vi "VI Doc Editor.vi"(11 "VI Path in":path) -> (0 "OK out":bool, 3 "dup VI Path in":path)   [LabVIEW 2014]
doc: "::: VI Helpeks :::\nCopyright (c) 2000-2026 Konstantin Shifershteyn. All rights reserved."
uses:
  <vilib>/event_ctls.llb/lveventtype.ctl
  <vilib>/Utility/miscctls.llb/LVPointTypeDef.ctl
  <vilib>/picture/picture.llb/imagedata.ctl
  <vilib>/Utility/cursorutil.llb/Set Cursor (Icon Pict).vi
  _VIH Support Library.llb/VIH Utility - APP - Is Value Changed (I32).vi
  _VIH Support Library.llb/VIH Utility - MENU - Create Menu (String).vi
panel:
  out "Conpane Image":picture caption="Connector Pane Image"
  in  "Ctrl Tree":string[](tree) caption="Control Tree"
  in  "Sort":cluster{"Column":i32, "Reverse":bool}
  in  "App Refnum":refnum<vi>
  in  "Good VI":bool
  in  "Changed":bool
  in  "VI Path":path
  in  "Tab Control":enum32{"VI Properties", "Control Properties"}(tab)
  out "VI Version":string caption="Source version"
  in  "VI Cust Title":bool caption="Same as VI Name"
  in  "VI Title":string caption="VI Front Panel Title"
  out "VI Icon":picture
  in  "VI Help Path":path caption="Help Path"
  in  "VI Help Tag":string caption="Help Tag"
  in  "VI Description":string
  in  "VI Help Use Url":i16(ring) caption="Help Used" items=["Local Help File", "Web-based Help"]
  in  "VI Help Url":string caption="Help URL"
  out "Ctrl Icon":picture caption="Terminal icon"
  in  "Ctrl Tooltip":string caption="Tip"
  in  "Ctrl Description":string caption="Description"
  in  "Ctrl Caption":string caption="Caption"
  out "Ctrl Label":string="Control label" caption="Control Label"
  in  "ConpaneMenuActive":bool
  in  "%OpenVI":bool caption="Open VI"
  in  "%Apply&Save":bool caption="Apply and Save VI"
  in  "%Apply":bool caption="Apply to VI"
  in  "%EXIT":bool caption="Exit"
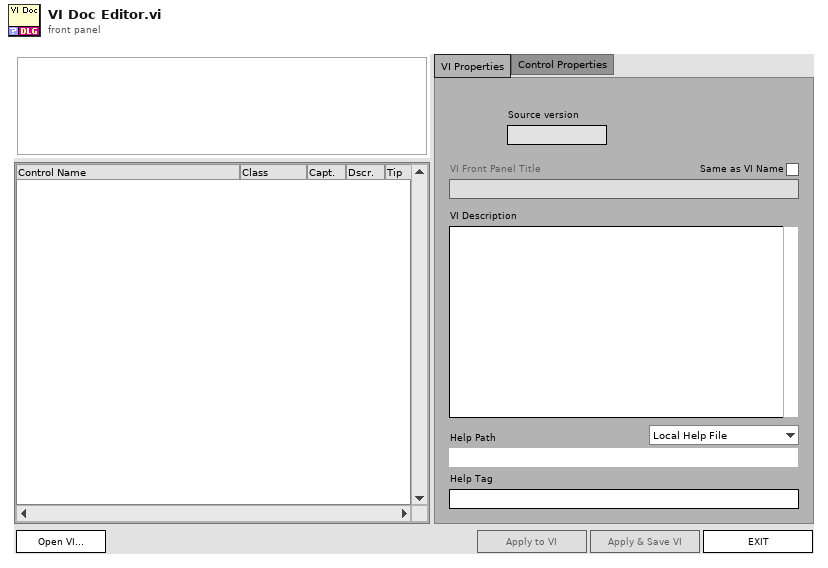
[diagram p1: front panel]
types:
  T1 = typedef "lveventtype.ctl" = enum32{"Null", "Timeout", "Annotation Menu Selection", "Annotation Menu Selection?", "App Instance Close", "App Instance Close?", "Autoscale Range Change", "Bookmark Info Change", "Cell Edit", "Cell Edit?", "Cursor Grab", "Cursor Grab?", "Cursor Menu Selection", "Cursor Menu Selection?", "Cursor Move", "Cursor Release", "Data Change", "Direction Change", "Display State Change", "Drag Ended", "Drag Enter", "Drag Leave", "Drag Over", "Drag Source Update", "Drag Starting", "Drag Starting?", "Drop", "Exec State Change", "Key Down", "Key Down?", "Key Repeat", "Key Repeat?", "Key Up", "Listbox Double Click", "Menu Activation?", "Menu Selection (App)", "Menu Selection? (App)", "Menu Selection (User)", "Mouse Down", "Mouse Down?", "Mouse Enter", "Mouse Leave", "Mouse Move", "Mouse Up", "Mouse Wheel", "NI Security User Change (App)", "Pane Size", "Panel Close", "Panel Close?", "Panel Resize", "Plot Attribute Change", "Scale Range Change", "Shortcut Menu Activation?", "Shortcut Menu Selection (App)", "Shortcut Menu Selection? (App)", "Shortcut Menu Selection (User)", "Tree Double Click", "Tree Drag", "Tree Drag?", "Tree Drop", "Tree Drop?", "Tree Item Close", "Tree Item Close?", "Tree Item Open", "Tree Item Open?", "User Event", "Value Change"}
  T2 = enum16{"nop", "Init", "get index", "get symbols"}
  T3 = typedef "LVPointTypeDef.ctl" = cluster{"Horizontal":i16, "Vertical":i16}
  T4 = cluster{"Width":i16, "Style":enum32{"Solid", "Dash", "Dot", "DashDot", "DashDotDot"}}
  T5 = enum16{"Apply", "ApplySave", "Continue", "Cancel"}
  T6 = typedef "imagedata.ctl" = cluster{"image type":i32, "image depth":i32, "image":u8[], "mask":u8[], "colors":u32[], "Rectangle":cluster{"left":i16, "top":i16, "right":i16, "bottom":i16}}
  T7 = cluster{"VI Reference":refnum<vi>, "Changed":bool, "Description":string, "Help.Path":path, "Help.Tag":string, "CustomTitle":bool, "Title":string, "Icon":T6, "Help.UseWebUrl":bool, "Help.WebUrl":string}
  T8 = enum32{"Bad", "Idle", "Run top level", "Running"}
  T9 = enum32{"Invalid", "Default", "Floating", "Floating/Auto-Hide", "Modal"}
  T10 = enum8{"Enabled", "Disabled", "Disabled and Grayed Out"}
  T11 = typedef "LVRectTypeDef.ctl" = cluster{"Left":i16, "Top":i16, "Right":i16, "Bottom":i16}
  T12 = typedef "LVPoint32TypeDef.ctl" = cluster{"Horizontal":i32, "Vertical":i32}
  T13 = typedef "LVMouseTypeDef.ctl" = cluster{"Mouse Position":cluster{"X":i32, "Y":i32}, "Mouse Modifiers":cluster{"Button Down":bool, "Shift Mod":bool, "Menu Mod":bool, "Option Mod":bool}}
  T14 = cluster{"Button Down":bool, "Shift Mod":bool, "Menu Mod":bool, "Option Mod":bool}
  T15 = cluster{"Ctrl ID":string, "Conpane Idx":i32, "Bounds":cluster{"X0":i32, "Y0":i32, "X1":i32, "Y1":i32}}[]
  T16 = cluster{"Ctrl ID":string, "Conpane Idx":i32, "Bounds":cluster{"X0":i32, "Y0":i32, "X1":i32, "Y1":i32}}
  T17 = typedef "VIH Project Tree Typedef - Tree Refnum.ctl" = refnum<vi>
  T18 = typedef "VIH - VI Doc Editor #2 Typedef - Info Cluster.ctl" = cluster{"Control Label":string, "Class Name":string, "Indicator":bool, "Error Cluster":bool, "Tree Tag":string, "Control ID":string, "Conpane Idx":i32, "Ctl Refnum":refnum<vi>, "Ctl Caption":string, "Ctl Description":string, "Ctl Tooltip":string, "Page Refnum":refnum<vi>}
  T19 = cluster{"Has Caption":bool, "Caption":string, "Description":string, "Tip Strip":string}
  T20 = cluster{"left":i16, "top":i16, "right":i16, "bottom":i16}
  T21 = typedef "LVBoundsTypeDef.ctl" = cluster{"Width":u32, "Height":u32}
  T22 = cluster{"image":picture, "Rectangle":cluster{"left":i16, "top":i16, "right":i16, "bottom":i16}}
  T23 = typedef "VIH HelpGen Typedef - Control Terminal Attributes Cluster.ctl" = cluster{"Conpane Idx":i32, "Control":bool, "Wire Rule":enum16{"Invalid Wire Rule", "Required", "Recommended", "Optional", "Dynamic Dispatch"}}
  T24 = cluster{"Description":string, "Help.Path":path, "Help.Tag":string, "CustomTitle":bool, "Title":string, "Help.UseWebUrl":bool, "Help.WebUrl":string}
  T25 = cluster{"Ctl Caption":string, "Ctl Description":string, "Ctl Tooltip":string}
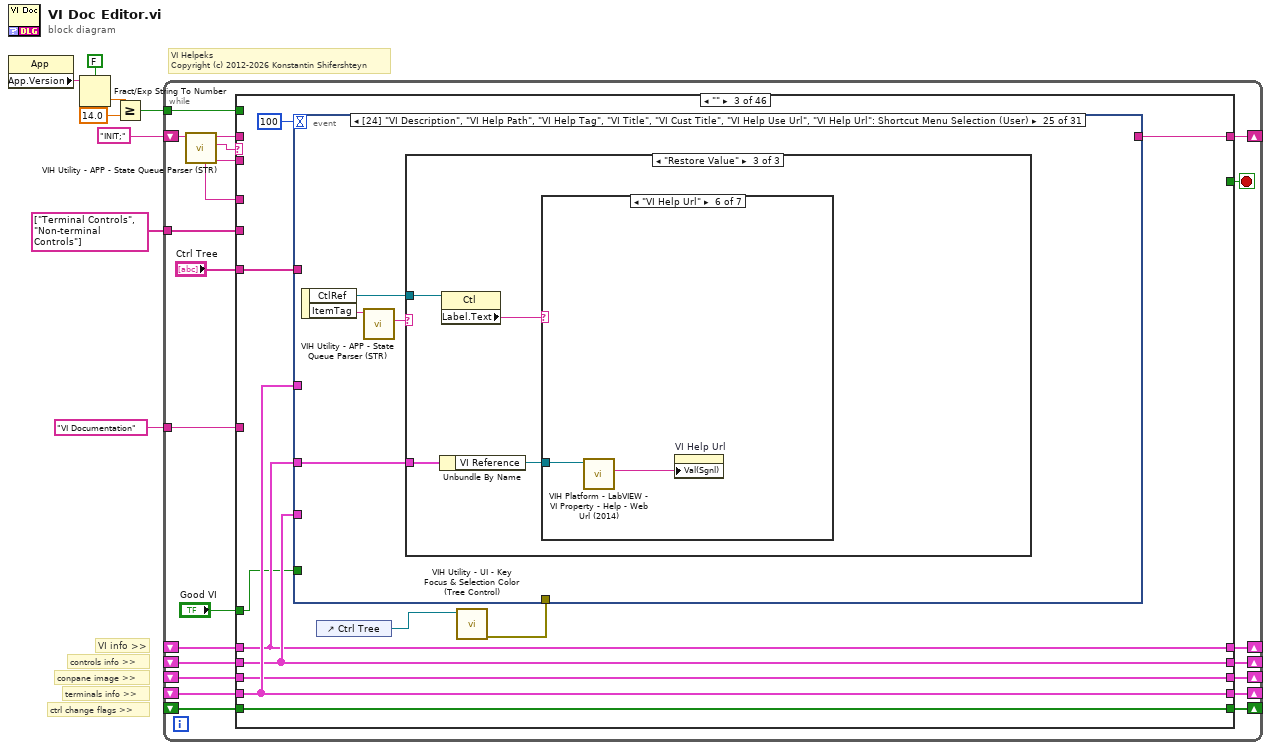
[diagram p0: block diagram]
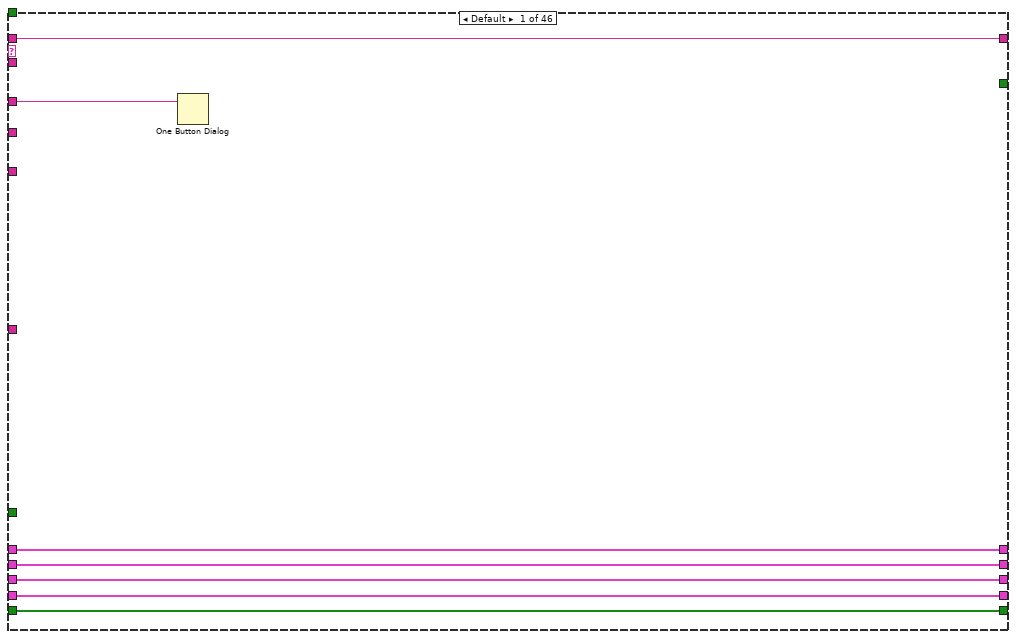
[diagram p2: hidden frame]
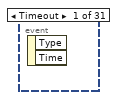
[diagram p4: hidden frame]
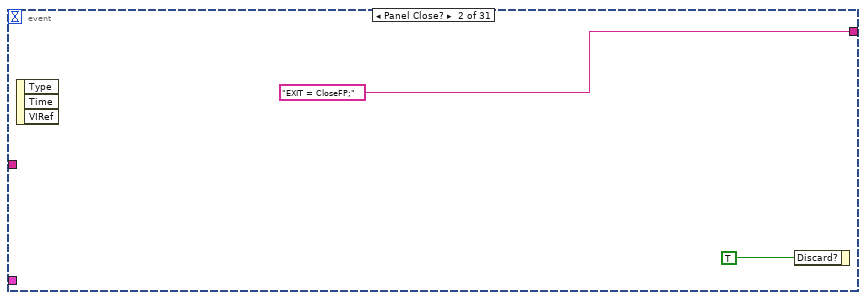
[diagram p5: hidden frame]
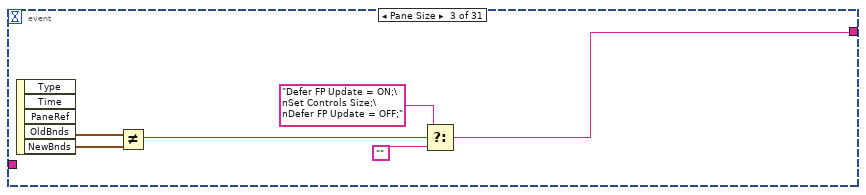
[diagram p6: hidden frame]
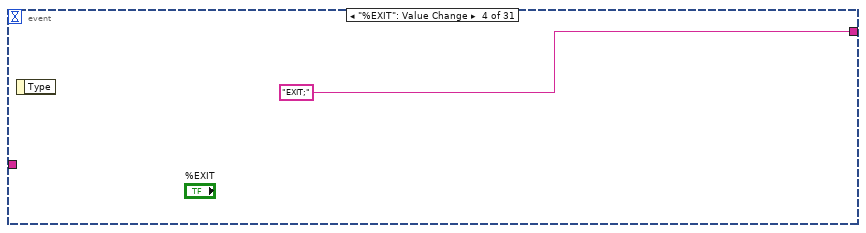
[diagram p7: hidden frame]
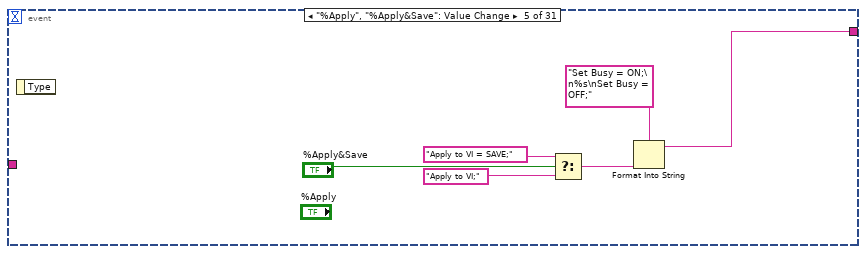
[diagram p8: hidden frame]
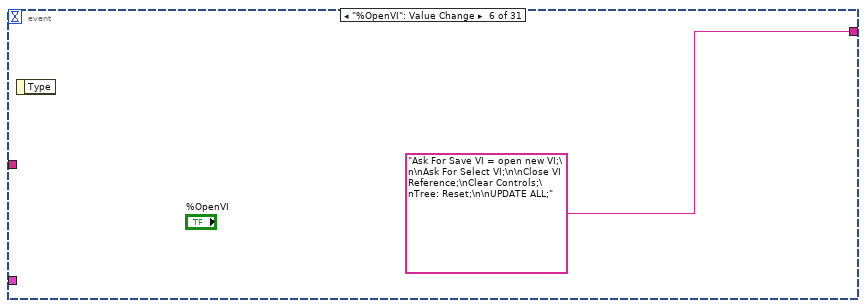
[diagram p9: hidden frame]
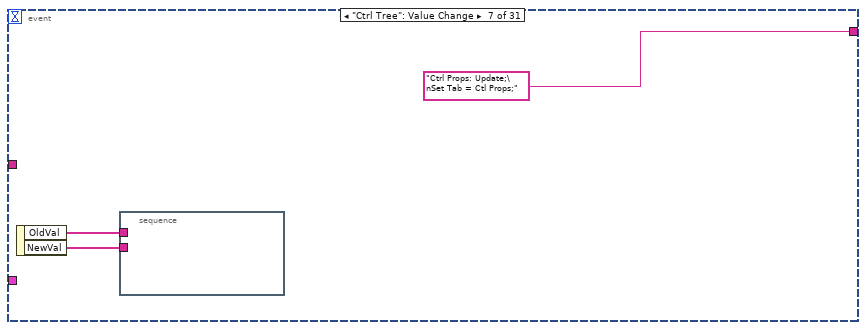
[diagram p10: hidden frame]
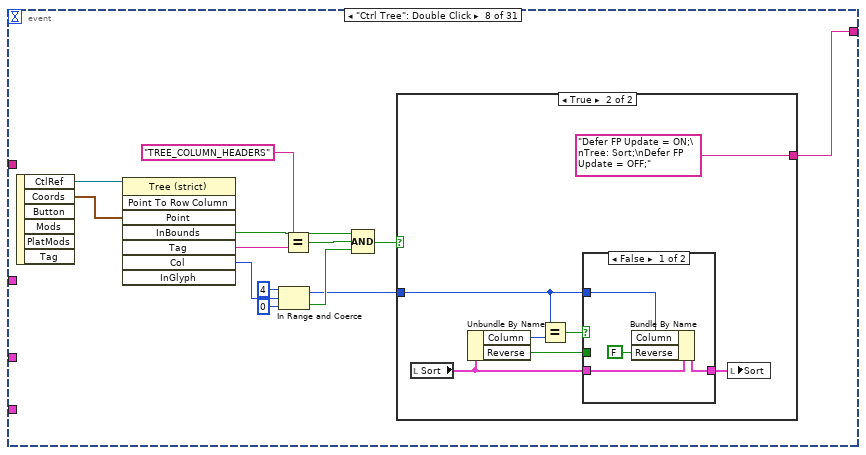
[diagram p11: hidden frame]
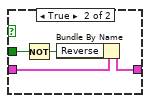
[diagram p13: hidden frame]
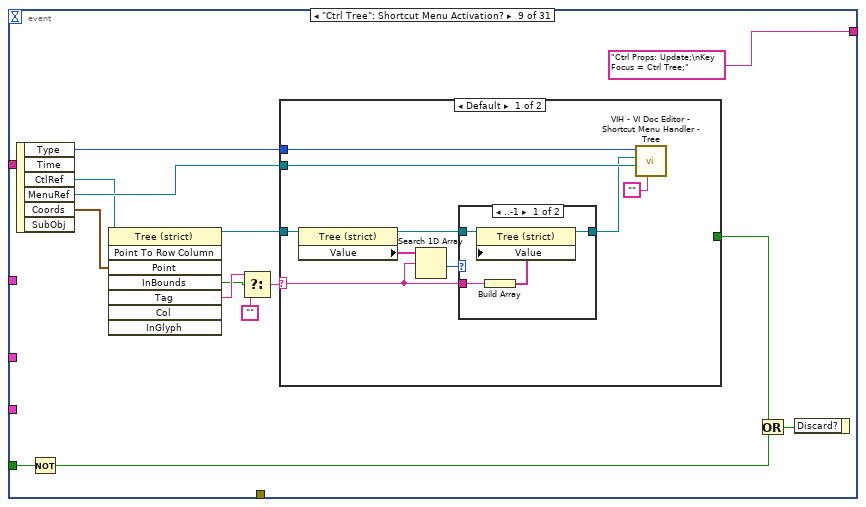
[diagram p14: hidden frame]
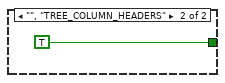
[diagram p16: hidden frame]
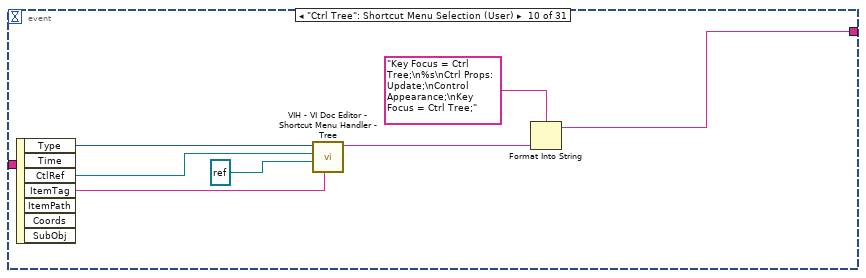
[diagram p17: hidden frame]
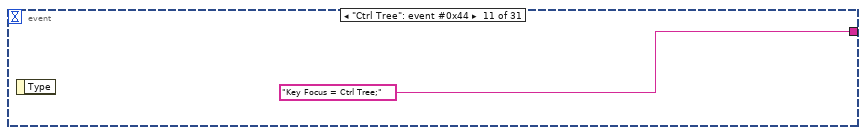
[diagram p18: hidden frame]
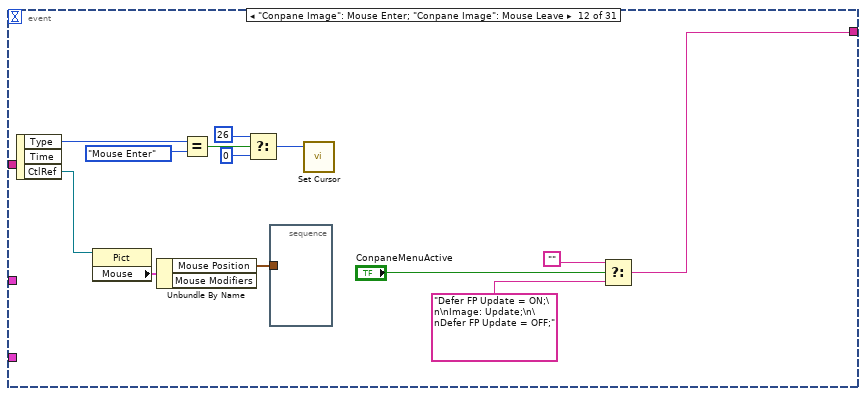
[diagram p19: hidden frame]
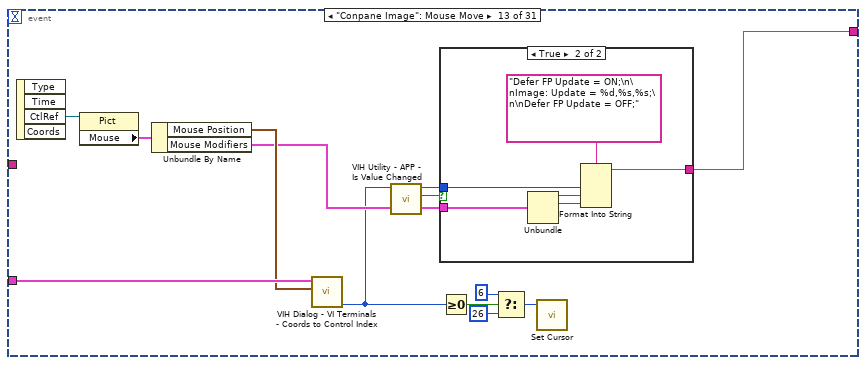
[diagram p20: hidden frame]
diagram:
  # "VI Helpeks\nCopyright (c) 2012-2026 Konstantin Shifershteyn"
  # "ctrl change flags >>"
  # "VI info >>"
  # "terminals info >>"
  # "conpane image >>"
  # "controls info >>"
  n1 = property class="App"() -> ("App.Version"=w6:string)  [unwired: 2 in, 2 out]
  n2 = Fract/Exp String To Number(use system decimal point (T)=FALSE, string=w6) -> (number=w4:dbl)  [unwired: 2 in, 1 out]
  n3 = Greater Or Equal?(x=w4, y=14.0) -> (x >= y?=w2:bool)
  n4 = while {
    shift-right: [w27] -> _
    shift-left: "INIT;" -> [w29]
    shift-right: [w22] -> _
    shift-left: _ -> [w21]
    shift-right: [w20] -> _
    shift-left: _ -> [w19]
    shift-right: [w18] -> _
    shift-left: _ -> [w17]
    tunnel: "VI Documentation" -> [w16]
    shift-right: [w15] -> _
    shift-left: _ -> [w14]
    shift-right: [w13] -> _
    shift-left: _ -> [w12]
    tunnel: w2 -> [w10]
    tunnel: string[] ["Terminal Controls", "Non-terminal Controls"] -> [w9]
    stop <- w23 stop-if-true
    n5 = call "VIH Utility - APP - State Queue Parser (STR).vi"("input queue"=w29) -> ("state parameters"=w25:string, "state"=w30:string, "remained queue"=w28:string, "complete state specifier"=w26:string)  [unwired: 5 in]
    n6 = case shown="\"\"" w30 {
      tunnel: w28 -> [w37 w43 _ w430 w466 _ w504 w512 w519 w528 w545 w587 w625 w633 w682 w685 w704 w709 w729 w760 w766 w800 w819 w861 w894 w935 w970 w997 w1021 w1028 w1035 w1042 w1055 w1108 w1112 w1158 w1188 w1208 w1229 w1250 w1262 w1318 w1347 w1367 w1389 w1556]
      tunnel: [w37 w43 w51 w427 w463 w468 w504 w512 w519 w528 w545 w587 w625 w633 w682 w684 w704 w708 w730 w760 w767 w800 w819 w861 w894 w935 w970 w997 w1021 w1028 w1035 w1042 w1055 w1108 w1112 w1158 w1188 w1202 w1225 w1250 w1262 w1309 w1346 w1367 w1378 w1550] -> w27
      tunnel: w26 -> [w36 _ _ _ _ _ _ _ _ _ _ _ _ _ _ _ _ _ _ _ _ _ _ _ _ _ _ _ _ _ _ _ _ _ _ _ _ _ _ _ _ _ _ _ _ _]
      tunnel: w25 -> [_ _ _ _ _ w467 w485 _ w518 w527 w544 _ _ w631 _ w689 _ _ w731 _ _ _ _ _ _ _ _ w982 _ _ _ _ w1047 _ _ _ _ _ w1221 _ w1258 w1305 w1342 _ w1380 w1547]
      tunnel: "Ctrl Tree" -> [_ _ w45 _ _ _ _ _ _ _ _ _ _ _ _ _ _ _ _ _ _ _ _ _ _ _ _ _ _ _ _ w1039 w1045 _ _ _ _ _ _ _ w1257 w1320 _ _ _ _]
      tunnel: [_ _ _ _ _ _ TRUE _ _ _ _ _ _ _ _ _ _ _ _ _ _ _ _ _ _ _ _ _ _ _ _ _ _ _ _ _ _ _ _ _ _ _ _ _ _ _] -> w23
      tunnel: [w35 w42 w50 w429 w465 w474 w501 w511 w517 w524 w540 w586 w624 w632 w681 w694 w703 w719 w737 w759 w783 w799 w818 w838 w893 w916 w968 w995 w1019 w1026 w1033 w1041 w1054 w1107 w1116 w1166 w1187 w1207 w1228 w1249 w1261 w1317 w1353 w1366 w1388 w1555] -> w22
      tunnel: w21 -> [w35 w42 w50 w429 w465 w474 w501 w511 w517 w524 w540 w586 w624 w632 w681 w694 w703 w719 w737 w759 w783 w799 w818 w838 w893 _ w968 w995 w1019 w1026 w1033 w1041 w1054 w1107 w1116 w1166 w1187 w1207 w1228 w1249 w1261 w1317 w1353 w1366 w1388 w1555]
      tunnel: [w34 w41 w49 w428 w464 w473 w500 w510 w516 w523 w539 w585 w623 w630 w680 w693 w702 w718 w736 w758 w782 w798 w817 w834 w892 w909 w969 w996 w1020 w1025 w1032 w1040 w1053 w1106 w1115 w1165 w1186 w1206 w1227 w1248 w1260 w1316 w1352 w1365 w1387 w1554] -> w20
      tunnel: w19 -> [w34 w41 w49 w428 w464 w473 w500 w510 w516 w523 w539 w585 w623 w630 w680 w693 w702 w718 w736 w758 w782 w798 w817 _ w892 w909 w969 w996 w1020 w1025 w1032 w1040 w1053 w1106 w1115 w1165 w1186 w1206 w1227 w1248 w1260 w1316 w1352 w1365 w1387 w1554]
      tunnel: [w33 w40 w48 w426 w462 w472 w497 w509 w515 w522 w534 w584 w622 w629 w679 w692 w701 w717 w735 w757 w781 w796 w816 w837 w891 w918 w967 w994 w1018 w1024 w1031 w1038 w1050 w1105 w1114 w1164 w1185 w1205 w1226 w1247 w1251 w1315 w1348 w1364 w1382 w1552] -> w18
      tunnel: w17 -> [w33 w40 w48 w426 w462 w472 w497 w509 w515 w522 w534 w584 w622 w629 w679 w692 w701 w717 w735 w757 w781 w796 w816 w837 w891 _ w967 w994 w1018 w1024 w1031 w1038 w1050 w1105 w1114 w1164 w1185 w1205 w1226 w1247 w1255 w1315 w1350 w1364 w1382 w1552]
      tunnel: w16 -> [_ _ _ _ _ _ w499 _ _ _ _ w583 _ _ _ _ _ _ w732 _ _ w797 _ _ _ _ _ _ _ _ _ _ _ _ _ _ _ _ _ _ _ _ _ _ _ _]
      tunnel: [w32 w39 w46 w423 w461 w471 w496 w508 w514 w521 w533 w580 w621 w628 w678 w691 w700 w716 w734 w756 w780 w793 w804 w841 w890 w924 w965 w993 w1017 w1023 w1030 w1037 w1052 w1104 w1110 w1157 w1184 w1203 w1223 w1246 w1259 w1314 w1351 w1363 w1384 w1553] -> w15
      tunnel: w14 -> [w32 w39 w46 w423 w461 w471 w496 w508 w514 w521 w533 w580 w621 w628 w678 w691 w700 w716 w734 w756 _ w793 w804 w841 w890 w924 w965 w993 w1017 w1023 w1030 w1037 w1052 w1104 w1111 w1156 w1184 w1204 w1220 w1246 w1259 w1314 w1351 w1363 w1384 w1553]
      tunnel: [w31 w38 w47 w422 w460 w470 w495 w507 w513 w520 w532 w579 w616 w627 w677 w690 w699 w715 w733 w755 w779 w791 w815 w839 w889 w910 w962 w992 w1016 w1022 w1029 w1036 w1048 w1103 w1113 w1159 w1181 w1200 w1224 w1245 w1252 w1307 w1345 w1362 w1381 w1551] -> w13
      tunnel: w12 -> [w31 w38 w47 w422 w460 w470 w495 w507 w513 w520 w532 w579 w616 w627 w677 w690 w699 w715 w733 w755 w779 w791 w815 w839 w889 _ w962 w992 w1016 w1022 w1029 w1036 w1049 w1103 w1113 w1159 w1181 w1200 w1224 w1245 w1253 w1307 w1345 w1362 w1381 w1551]
      tunnel: "Good VI" -> [_ _ w44 _ _ _ _ _ _ _ _ w574 _ _ _ _ _ _ _ _ _ _ _ w833 _ _ _ _ _ _ _ _ _ _ _ _ w1173 _ _ _ _ w1304 _ _ _ _]
      tunnel: w10 -> [_ _ _ w406 _ _ _ _ _ _ _ _ _ _ _ _ _ _ _ _ _ _ _ _ _ _ _ _ _ _ _ _ _ _ _ _ w1167 _ _ _ _ _ _ _ _ _]
      tunnel: w9 -> [_ _ _ _ _ _ _ _ _ _ _ _ _ _ _ _ _ _ _ _ _ _ _ _ _ w895 w960 w976 _ _ _ _ _ _ _ _ _ _ _ _ _ _ _ _ _ _]
      frame Default {
        n7 = One Button Dialog(message=w36) -> ()  [unwired: 1 in, 1 out]
      }
      frame "#" {
      }
      frame "" {
        n8 = control-ref of="Ctrl Tree"() -> (w53:refnum<vi>)
        n9 = call "VIH Utility - UI - Key Focus & Selection Color (Tree Control).vi"("Tree Refnum"=w53) -> ("error out"=w52:errorcluster)  [unwired: 8 in, 2 out]
        n10 = event shown="[24] \"VI Description\", \"VI Help Path\", \"VI Help Tag\", \"VI Title\", \"VI Cust Title\", \"VI Help Use Url\", \"VI Help Url\": Shortcut Menu Selection (User)" {
          selector: _ -> [_ _ _ _ _ _ _ _ _ _ _ _ _ _ _ _ _ _ _ _ _ _ _ _ _ _ _ _ _ _ _]
          dyn-events: _ -> [_ _ _ _ _ _ _ _ _ _ _ _ _ _ _ _ _ _ _ _ _ _ _ _ _ _ _ _ _ _ _]
          timeout: 100 -> [_ _ _ _ _ _ _ _ _ _ _ _ _ _ _ _ _ _ _ _ _ _ _ _ _ _ _ _ _ _ _]
          tunnel: w52 -> [_ _ _ _ _ _ _ _ _ _ _ _ _ _ _ _ _ _ _ _ _ _ _ _ _ _ _ _ _ _ _]
          tunnel: [_ "EXIT = CloseFP;" w57 "EXIT;" w64 "Ask For Save VI = open new VI;\n\nAsk For Select VI;\n\nClose VI Reference;\nClear Controls;\nTree: Reset;\n\nUPDATE ALL;" "Ctrl Props: Update;\nSet Tab = Ctl Props;" w74 "Ctrl Props: Update;\nKey Focus = Ctrl Tree;" w132 "Key Focus = Ctrl Tree;" w142 w160 w176 w196 w263 w291 "Key Focus = Ctrl Tree;" "Image: Update;" "Image: Update;" w315 "VI Props: Apply;" _ _ _ w358 _ _ _ _ w395] -> w51
          tunnel: w50 -> [_ _ _ _ _ _ _ _ _ _ _ _ w164 w178 w199 w269 w288 w303 _ _ w316 _ _ _ _ _ _ _ _ _ _]
          tunnel: w48 -> [_ _ _ _ _ _ _ _ _ _ _ _ _ _ w190 w247 w275 _ _ _ _ _ _ _ _ _ _ w363 _ _ _]
          tunnel: w46 -> [_ _ _ _ _ _ _ _ _ _ _ _ _ _ _ _ _ _ _ _ _ _ _ _ w330 _ _ w367 _ _ _]
          tunnel: w45 -> [_ _ _ _ _ _ _ _ _ _ _ _ _ _ _ _ _ _ _ _ _ _ _ _ _ w360 _ w364 _ _ _]
          tunnel: w44 -> [_ _ _ _ _ _ _ _ w105 _ _ _ _ _ _ w244 _ _ _ _ _ _ _ _ _ _ _ _ _ _ _]
          event Timeout {
            n11 = event-data() -> ()  [unwired: 1 in, 2 out]
          }
          event Panel Close? {
            n12 = event-data() -> ()  [unwired: 1 in, 3 out]
            n13 = event-data("Discard?"=TRUE) -> ()  [unwired: 1 in, 1 out]
          }
          event Pane Size {
            n14 = event-data() -> ("OldBnds"=w62:T11, "NewBnds"=w61:T11)  [unwired: 1 in, 3 out]
            n15 = Not Equal?(x=w62, y=w61) -> (x != y?=w60:bool)
            n16 = Select(t="Defer FP Update = ON;\nSet Controls Size;\nDefer FP Update = OFF;", s=w60, f="") -> (s? t:f=w57:string)
          }
          event "%EXIT": Value Change {
            n17 = event-data() -> ()  [unwired: 1 in, 1 out]
          }
          event "%Apply", "%Apply&Save": Value Change {
            n18 = event-data() -> ()  [unwired: 1 in, 1 out]
            n19 = Select(t="Apply to VI = SAVE;", s="%Apply&Save", f="Apply to VI;") -> (s? t:f=w66:string)
            n20 = Format Into String(format string="Set Busy = ON;\n%s\nSet Busy = OFF;", w66) -> (resulting string=w64:string)  [unwired: 2 in, 1 out]
          }
          event "%OpenVI": Value Change {
            n21 = event-data() -> ()  [unwired: 1 in, 1 out]
          }
          event "Ctrl Tree": Value Change {
            n22 = event-data() -> ("OldVal"=w72:string[], "NewVal"=w71:string[])  [unwired: 1 in]
            n23 = stacked-sequence {
              tunnel: w72 -> [_]
              tunnel: w71 -> [_]
              frame #0 {
              }
            }
          }
          event "Ctrl Tree": Double Click {
            n24 = event-data() -> ("CtlRef"=w86:refnum<vi>, "Coords"=w85:T12)  [unwired: 1 in, 4 out]
            n25 = invoke class="Tree (strict)" method="Point To Row Column"(reference=w86, "Point"=w85) -> ("InBounds"=w79:bool, "Tag"=w81:string, "Col"=w84:i32)  [unwired: 6 in, 5 out]
            n26 = In Range and Coerce(upper limit=4, x=w84, lower limit=0) -> (coerced(x)=w75:i32, In Range?=w77:bool)
            n27 = Equal?(x="TREE_COLUMN_HEADERS", y=w81) -> (x = y?=w78:bool)
            n28 = Compound Arithmetic op=AND(w79, w78, w77) -> (w76:bool)
            n29 = case shown="True" w76 {
              tunnel: w75 -> [_ w88]
              tunnel: [_ "Defer FP Update = ON;\nTree: Sort;\nDefer FP Update = OFF;"] -> w74
              frame False {
              }
              frame True {
                n30 = local read "Sort"() -> (w92:cluster{"Column":i32, "Reverse":bool})
                n31 = Unbundle By Name(w92) -> ("Column"=w89:i32, "Reverse"=w91:bool)
                n32 = Equal?(x=w88, y=w89) -> (x = y?=w93:bool)
                n33 = case shown="False" w93 {
                  tunnel: w92 -> [w97 w101]
                  tunnel: w91 -> [_ w100]
                  tunnel: [w96 w99] -> w90
                  tunnel: w88 -> [w94 _]
                  frame False {
                    n34 = Bundle By Name(cluster=w97, "Column"=w94, "Reverse"=FALSE) -> (w96:cluster{"Column":i32, "Reverse":bool})
                  }
                  frame True {
                    n35 = Not(x=w100) -> (.not. x?=w98:bool)
                    n36 = Bundle By Name(cluster=w101, "Reverse"=w98) -> (w99:cluster{"Column":i32, "Reverse":bool})
                  }
                }
                n37 = local write "Sort"(w90) -> ()
              }
            }
          }
          event "Ctrl Tree": Shortcut Menu Activation? {
            n38 = event-data() -> ("Type"=w109:T1, "CtlRef"=w106:refnum<vi>, "MenuRef"=w108:refnum<k9>, "Coords"=w107:T12)  [unwired: 1 in, 2 out]
            n39 = Not(x=w105) -> (.not. x?=w104:bool)
            n40 = invoke class="Tree (strict)" method="Point To Row Column"(reference=w106, "Point"=w107) -> (reference out=w114:refnum<vi>, "InBounds"=w110:bool, "Tag"=w111:string)  [unwired: 6 in, 5 out]
            n41 = Select(t=w111, s=w110, f="") -> (s? t:f=w113:string)
            n42 = case shown="Default" w113 {
              selector: w113 -> [w119 _]
              tunnel: w108 -> [w120 _]
              tunnel: [_ TRUE] -> w103
              tunnel: w114 -> [w117 _]
              tunnel: w109 -> [w121 _]
              frame Default {
                n43 = property class="Tree (strict)"(reference=w117) -> (reference out=w122:refnum<vi>, "Value"=w124:string[])  [unwired: 1 in, 1 out]
                n44 = Search 1D Array(1D array=w124, element=w119) -> (index of element=w123:i32)  [unwired: 1 in]
                n45 = case shown="..-1" w123 {
                  tunnel: w122 -> [w128 w129]
                  tunnel: w119 -> [w127 _]
                  tunnel: [w125 w129] -> w116
                  frame ..-1 {
                    n46 = Build Array(w127) -> (w126:string[])
                    n47 = property class="Tree (strict)"(reference=w128, "Value"=w126) -> (reference out=w125:refnum<vi>)  [unwired: 1 in, 1 out]
                  }
                  frame 0.. {
                  }
                }
                n48 = call "VIH - VI Doc Editor - Shortcut Menu Handler - Tree.vi"("Menu Tag"="", "MenuRef"=w120, "Terminals Tree"=w116, "Event Type"=w121) -> ()  [unwired: 7 in, 1 out]
              }
              frame "", "TREE_COLUMN_HEADERS" {
              }
            }
            n49 = Or(x=w103, y=w104) -> (x .or. y?=w102:bool)
            n50 = event-data("Discard?"=w102) -> ()  [unwired: 1 in, 1 out]
          }
          event "Ctrl Tree": Shortcut Menu Selection (User) {
            n51 = event-data() -> ("Type"=w136:T1, "CtlRef"=w135:refnum<vi>, "ItemTag"=w134:string)  [unwired: 1 in, 4 out]
            n52 = call "VIH - VI Doc Editor - Shortcut Menu Handler - Tree.vi"("Menu Tag"=w134, "MenuRef"=refnum<k9> refnum, "Terminals Tree"=w135, "Event Type"=w136) -> ("States spec"=w133:string)  [unwired: 7 in]
            n53 = Format Into String(format string="Key Focus = Ctrl Tree;\n%s\nCtrl Props: Update;\nControl Appearance;\nKey Focus = Ctrl Tree;", w133) -> (resulting string=w132:string)  [unwired: 2 in, 1 out]
          }
          event "Ctrl Tree": event #0x44 {
            n54 = event-data() -> ()  [unwired: 1 in, 1 out]
          }
          event "Conpane Image": Mouse Enter; "Conpane Image": Mouse Leave {
            n55 = event-data() -> ("Type"=w151:T1, "CtlRef"=w140:refnum<vi>)  [unwired: 1 in, 1 out]
            n56 = property on="Property Node" class="Pict"(reference=w140) -> ("Mouse"=w141:T13)  [unwired: 1 in, 2 out]
            n57 = Unbundle By Name(w141) -> ("Mouse Position"=w139:cluster{"X":i32, "Y":i32})  [unwired: 1 out]
            n58 = Equal?(x=w151, y=lveventtype."Mouse Enter" ("Type")) -> (x = y?=w149:bool)
            n59 = Select(t=u16 26 ("icon"), s=w149, f=u16 0) -> (s? t:f=w146:u16)
            n60 = stacked-sequence {
              tunnel: w139 -> [_]
              frame #0 {
              }
            }
            n61 = call-poly <vilib>:"Set Cursor.vi"("icon"=w146) -> ()  [unwired: 9 in, 2 out]
            n62 = Select(t="", s="ConpaneMenuActive", f="Defer FP Update = ON;\n\nImage: Update;\n\nDefer FP Update = OFF;") -> (s? t:f=w142:string)
          }
          event "Conpane Image": Mouse Move {
            n63 = event-data() -> ("CtlRef"=w163:refnum<vi>)  [unwired: 1 in, 3 out]
            n64 = property on="Property Node" class="Pict"(reference=w163) -> ("Mouse"=w162:T13)  [unwired: 1 in, 2 out]
            n65 = Unbundle By Name(w162) -> ("Mouse Position"=w161:cluster{"X":i32, "Y":i32}, "Mouse Modifiers"=w157:T14)
            n66 = call "VIH Dialog - VI Terminals - Coords to Control Index.vi"("Coords"=w161, "Controls info"=w164) -> ("Index"=w152:i32)  [unwired: 8 in, 1 out]
            n67 = call-poly "VIH Utility - APP - Is Value Changed.vi"("Value"=w152) -> ("Changed"=w158:bool, "dup Value"=w159:i32)  [unwired: 5 in]
            n68 = case shown="True" w158 {
              tunnel: [_ w169] -> w160
              tunnel: w159 -> [_ w168]
              tunnel: w157 -> [_ w167]
              frame False {
              }
              frame True {
                n69 = Unbundle(w167) -> ("Button Down"=w166:bool, "Shift Mod"=w165:bool)  [unwired: 2 out]
                n70 = Format Into String(format string="Defer FP Update = ON;\n\nImage: Update = %d,%s,%s;\n\nDefer FP Update = OFF;", w168, w166, w165) -> (resulting string=w169:string)  [unwired: 2 in, 1 out]
              }
            }
            n71 = Greater Or Equal To 0?(x=w152) -> (x >= 0?=w156:bool)
            n72 = Select(t=u16 6 ("icon"), s=w156, f=u16 26) -> (s? t:f=w155:u16)
            n73 = call-poly <vilib>:"Set Cursor.vi"("icon"=w155) -> ()  [unwired: 9 in, 2 out]
          }
          event "Conpane Image": Mouse Down {
            n74 = event-data() -> ("CtlRef"=w174:refnum<vi>, "Button"=w171:u16)  [unwired: 1 in, 5 out]
            n75 = property on="Property Node" class="Pict"(reference=w174) -> ("Mouse"=w175:T13)  [unwired: 1 in, 2 out]
            n76 = Unbundle By Name(w175) -> ("Mouse Position"=w173:cluster{"X":i32, "Y":i32}, "Mouse Modifiers"=w172:T14)
            n77 = case shown="1" w171 {
              tunnel: w178 -> [_ w182]
              tunnel: [-1 ("Index") w181] -> w177
              tunnel: w173 -> [_ w180]
              frame Default {
              }
              frame 1 {
                n78 = call "VIH Dialog - VI Terminals - Coords to Control Index.vi"("Coords"=w180, "Controls info"=w182) -> ("Index"=w181:i32)  [unwired: 8 in, 1 out]
              }
            }
            n79 = case shown="0.." w177 {
              selector: w177 -> [_ w188]
              tunnel: ["Key Focus = Ctrl Tree;" w187] -> w176
              tunnel: w172 -> [_ w185]
              frame ..-1 {
              }
              frame 0.. {
                n80 = Unbundle(w185) -> ("Button Down"=w184:bool, "Shift Mod"=w186:bool)  [unwired: 2 out]
                n81 = Format Into String(format string="Image: Update = %d,%s,%s;\nKey Focus = Ctrl Tree;", w188, w184, w186) -> (resulting string=w187:string)  [unwired: 2 in, 1 out]
              }
            }
          }
          event "Conpane Image": Mouse Up {
            n82 = event-data() -> ("CtlRef"=w194:refnum<vi>, "Button"=w191:u16)  [unwired: 1 in, 5 out]
            n83 = property on="Property Node" class="Pict"(reference=w194) -> ("Mouse"=w195:T13)  [unwired: 1 in, 2 out]
            n84 = Unbundle By Name(w195) -> ("Mouse Position"=w193:cluster{"X":i32, "Y":i32}, "Mouse Modifiers"=w192:T14)
            n85 = case shown="1" w191 {
              tunnel: w199 -> [w201 w205]
              tunnel: [w201 w204] -> w198
              tunnel: [-1 ("Index") w203] -> w197
              tunnel: w193 -> [_ w202]
              frame 0, Default {
              }
              frame 1 {
                n86 = call "VIH Dialog - VI Terminals - Coords to Control Index.vi"("Coords"=w202, "Controls info"=w205) -> ("Index"=w203:i32, "dup Controls info"=w204:T15)  [unwired: 8 in]
              }
            }
            n87 = case shown="0.." w197 {
              selector: w197 -> [_ w227]
              tunnel: w198 -> [_ w230]
              tunnel: ["Key Focus = Ctrl Tree;" w226] -> w196
              tunnel: w192 -> [_ w225]
              tunnel: w190 -> [_ w221]
              frame ..-1 {
                (unwired) "Image: Update;\nKey Focus = Ctrl Tree;"
              }
              frame 0.. {
                n88 = Index Array(array=w230, index=w227) -> (element=w229:T16)
                n89 = for {
                  tunnel: w221 -> [w235] mode=indexing
                  tunnel: [w233] -> w220 mode=indexing
                  tunnel: [w232] -> w216 mode=indexing
                  n90 = Unbundle By Name(w235) -> ("Tree Tag"=w232:string, "Control ID"=w234:string, "Conpane Idx"=w231:i32)
                  n91 = Bundle("Control ID"=w234, "Conpane Idx"=w231) -> (w233:cluster{"Control ID":string, "Conpane Idx":i32})  [unwired: 1 in]
                }
                n92 = Unbundle By Name(w229) -> ("Ctrl ID"=w219:string, "Conpane Idx"=w218:i32)
                n93 = control-ref of="Ctrl Tree"() -> (w211:refnum<vi>)
                n94 = Unbundle(w225) -> ("Button Down"=w224:bool, "Shift Mod"=w209:bool)  [unwired: 2 out]
                n95 = Bundle("Ctrl ID"=w219, "Conpane Idx"=w218) -> (w217:cluster{"Ctrl ID":string, "Conpane Idx":i32})  [unwired: 1 in]
                n96 = call "VIH Project Tree - Defer Panel Updates.vi"("Defer Panel Updates (F)"=TRUE, "Project Tree"=w211) -> ("error out"=w210:errorcluster, "dup Project Tree"=w212:T17)  [unwired: 7 in, 1 out]
                n97 = And(x=w209, y=FALSE) -> (x .and. y?=w208:bool)
                n98 = Search 1D Array(1D array=w220, element=w217) -> (index of element=w215:i32)  [unwired: 1 in]
                n99 = Index Array(array=w216, index=w215) -> (element=w214:string)
                n100 = case shown="True" w208 {
                  tunnel: [w236 w242] -> w223
                  tunnel: w212 -> [_ w241]
                  tunnel: w214 -> [w237 w240]
                  frame False {
                    n101 = Build Array(w237) -> (w236:string[])
                  }
                  frame True {
                    n102 = call "VIH Project Tree - Get Tree Item Tags.vi"("Parent Item Tag"=w240, "Project Tree"=w241) -> ("Child Item Tags"=w238:string[], "dup Parent Item Tag"=w239:string)  [unwired: 6 in, 2 out]
                    n103 = Build Array (concatenate)(w239, w238) -> (w242:string[])
                  }
                }
                n104 = invoke on="Ctrl Tree" class="Tree (strict)" method="Open/Close.Ensure Visible"(error in=w210, "tag"=w214) -> (error out=w222:errorcluster)  [unwired: 2 in, 3 out]
                n105 = Format Into String(format string="Tree: Open Items;\nCtrl Props: Update;\n\nDefer FP Update = OFF;\n\nImage: Update = %d,%s,%s;\nKey Focus = Ctrl Tree;", w227, w224, w209) -> (resulting string=w226:string)  [unwired: 2 in, 1 out]
                n106 = property on="Ctrl Tree" class="Tree (strict)"(error in=w222, "Val(Sgnl)"=w223) -> ()  [unwired: 1 in, 2 out]
              }
            }
          }
          event "Conpane Image": Shortcut Menu Activation? {
            n107 = event-data() -> ("Type"=w266:T1, "CtlRef"=w257:refnum<vi>, "MenuRef"=w264:refnum<k9>, "Coords"=w256:T12)  [unwired: 1 in, 1 out]
            n108 = Not(x=w244) -> (.not. x?=w243:bool)
            n109 = local write "ConpaneMenuActive"(TRUE ("ConpaneMenuActive")) -> ()
            n110 = call "VIH UI - Convert Pane Coords to Picture Control Coords.vi"("Pane Coords"=w256, "Pict Refnum"=w257) -> ("Picture Coords"=w255:cluster{"Horizontal":i32, "Vertical":i32})  [unwired: 8 in, 1 out]
            n111 = call "VIH Dialog - VI Terminals - Coords to Control Index.vi"("Coords"=w255, "Controls info"=w269) -> ("Index"=w268:i32, "dup Controls info"=w267:T15)  [unwired: 8 in]
            n112 = for {
              tunnel: w247 -> [w273] mode=indexing
              tunnel: [w271] -> w251 mode=indexing
              n113 = Unbundle By Name(w273) -> ("Control ID"=w272:string, "Conpane Idx"=w270:i32)
              n114 = Bundle("Control ID"=w272, "Conpane Idx"=w270) -> (w271:cluster{"Control ID":string, "Conpane Idx":i32})  [unwired: 1 in]
            }
            n115 = Index Array(array=w267, index=w268) -> (element=w246:T16)
            n116 = Unbundle By Name(w246) -> ("Ctrl ID"=w250:string, "Conpane Idx"=w249:i32)
            n117 = Bundle("Ctrl ID"=w250, "Conpane Idx"=w249) -> (w248:cluster{"Ctrl ID":string, "Conpane Idx":i32})  [unwired: 1 in]
            n118 = control-ref of="Ctrl Tree"() -> (w265:refnum<vi>)
            n119 = Search 1D Array(1D array=w251, element=w248) -> (index of element=w245:i32)  [unwired: 1 in]
            n120 = Index Array(array=w247, index=w245) -> (element=w254:T18)
            n121 = Unbundle By Name(w254) -> ("Tree Tag"=w252:string, "Class Name"=w253:string)
            n122 = Format Into String(format string="Image: Update = %d,%s,%s;\nKey Focus = Ctrl Tree;", w268, FALSE, FALSE) -> (resulting string=w263:string)  [unwired: 2 in, 1 out]
            n123 = call "VIH - VI Doc Editor - Shortcut Menu Handler - Picture.vi"("Class Name"=w253, "Menu Tag"="", "Tree Item Tag"=w252, "MenuRef"=w264, "Terminals Tree"=w265, "Event Type"=w266) -> ()  [unwired: 5 in, 1 out]
            n124 = event-data("Discard?"=w243) -> ()  [unwired: 1 in, 1 out]
          }
          event "Conpane Image": Shortcut Menu Selection (User) {
            n125 = event-data() -> ("Type"=w296:T1, "CtlRef"=w284:refnum<vi>, "ItemTag"=w289:string, "Coords"=w285:T12)  [unwired: 1 in, 3 out]
            n126 = call "VIH UI - Convert Pane Coords to Picture Control Coords.vi"("Pane Coords"=w285, "Pict Refnum"=w284) -> ("Picture Coords"=w283:cluster{"Horizontal":i32, "Vertical":i32})  [unwired: 8 in, 1 out]
            n127 = control-ref of="Ctrl Tree"() -> (w295:refnum<vi>)
            n128 = call "VIH Dialog - VI Terminals - Coords to Control Index.vi"("Coords"=w283, "Controls info"=w288) -> ("Index"=w286:i32, "dup Controls info"=w287:T15)  [unwired: 8 in]
            n129 = for {
              tunnel: w275 -> [w300] mode=indexing
              tunnel: [w298] -> w280 mode=indexing
              n130 = Unbundle By Name(w300) -> ("Control ID"=w299:string, "Conpane Idx"=w297:i32)
              n131 = Bundle("Control ID"=w299, "Conpane Idx"=w297) -> (w298:cluster{"Control ID":string, "Conpane Idx":i32})  [unwired: 1 in]
            }
            n132 = Index Array(array=w287, index=w286) -> (element=w276:T16)
            n133 = Unbundle By Name(w276) -> ("Ctrl ID"=w279:string, "Conpane Idx"=w278:i32)
            n134 = Bundle("Ctrl ID"=w279, "Conpane Idx"=w278) -> (w277:cluster{"Ctrl ID":string, "Conpane Idx":i32})  [unwired: 1 in]
            n135 = Search 1D Array(1D array=w280, element=w277) -> (index of element=w274:i32)  [unwired: 1 in]
            n136 = Index Array(array=w275, index=w274) -> (element=w282:T18)
            n137 = Unbundle By Name(w282) -> ("Tree Tag"=w281:string)
            n138 = call "VIH - VI Doc Editor - Shortcut Menu Handler - Picture.vi"("Menu Tag"=w289, "Tree Item Tag"=w281, "MenuRef"=refnum<k9> refnum, "Terminals Tree"=w295, "Event Type"=w296) -> ("States spec"=w292:string)  [unwired: 6 in]
            n139 = local write "ConpaneMenuActive"(FALSE ("ConpaneMenuActive")) -> ()
            n140 = Format Into String(format string="Key Focus = Ctrl Tree;\n\n%s\nCtrl Props: Update;\nControl Appearance;\n\nDefer FP Update = OFF;\nKey Focus = Ctrl Tree;", w292) -> (resulting string=w291:string)  [unwired: 2 in, 1 out]
          }
          event "Conpane Image": event #0x44 {
            (unwired) "Image: Update;\nKey Focus = Ctrl Tree;"
            n141 = event-data() -> ("CtlRef"=w304:refnum<vi>)  [unwired: 1 in, 2 out]
            n142 = property on="Property Node" class="Pict"(reference=w304) -> ("Mouse"=w305:T13)  [unwired: 1 in, 2 out]
            n143 = Unbundle By Name(w305) -> ("Mouse Position"=w302:cluster{"X":i32, "Y":i32})  [unwired: 1 out]
            n144 = local write "ConpaneMenuActive"(FALSE ("ConpaneMenuActive")) -> ()
            n145 = call "VIH Dialog - VI Terminals - Coords to Control Index.vi"("Coords"=w302, "Controls info"=w303) -> ("Index"=w301:i32)  [unwired: 8 in, 1 out]
            n146 = stacked-sequence {
              tunnel: w301 -> [_]
              frame #0 {
              }
            }
          }
          event Mouse Enter {
            n147 = event-data() -> ()  [unwired: 1 in, 3 out]
          }
          event Mouse Down {
            n148 = event-data() -> ()  [unwired: 1 in, 1 out]
          }
          event Key Down; Key Up {
            n149 = event-data() -> ()  [unwired: 1 in, 7 out]
            n150 = property on="Conpane Image" class="Pict"() -> ("Mouse"=w314:T13)  [unwired: 2 in, 2 out]
            n151 = Unbundle By Name(w314) -> ("Mouse Position"=w313:cluster{"X":i32, "Y":i32}, "Mouse Modifiers"=w312:T14)
            n152 = call "VIH Dialog - VI Terminals - Coords to Control Index.vi"("Coords"=w313, "Controls info"=w316) -> ("Index"=w311:i32)  [unwired: 8 in, 1 out]
            n153 = case shown="0.." 0 ("Index") {
              tunnel: [_ w321] -> w315
              tunnel: w312 -> [_ w319]
              tunnel: w311 -> [_ w317]
              frame ..-1 {
              }
              frame 0.. {
                n154 = Unbundle(w319) -> ("Button Down"=w318:bool, "Shift Mod"=w320:bool)  [unwired: 2 out]
                n155 = Format Into String(format string="Image: Update = %d,%s,%s;", w317, w318, w320) -> (resulting string=w321:string)  [unwired: 2 in, 1 out]
              }
            }
          }
          event "VI Description", "VI Help Path", "VI Help Tag", "VI Title", "VI Cust Title", "VI Help Use Url", "VI Help Url": Value Change {
            n156 = event-data() -> ()  [unwired: 1 in, 1 out]
          }
          event "VI Description", "VI Help Tag", "VI Title", "VI Cust Title", "VI Help Use Url", "VI Help Url": Shortcut Menu Activation? {
            n157 = event-data() -> ("MenuRef"=w325:refnum<k9>)  [unwired: 1 in, 1 out]
            n158 = call-poly "VIH Utility - MENU - Create Menu.vi"("Menu Description"="Re-read from VI   | Restore Value", "menu"=w325) -> ()  [unwired: 8 in, 2 out]
            n159 = event-data() -> ()  [unwired: 2 in, 1 out]
          }
          event "VI Help Path": Shortcut Menu Activation? {
            n160 = event-data() -> ("MenuRef"=w327:refnum<k9>)  [unwired: 1 in, 1 out]
            n161 = call-poly "VIH Utility - MENU - Create Menu.vi"("Menu Description"="Browse for file...  | Select Help File\n--\nRe-read from VI     | Restore Value", "menu"=w327) -> ()  [unwired: 8 in, 2 out]
            n162 = event-data() -> ()  [unwired: 2 in, 1 out]
          }
          event "VI Description", "VI Help Path", "VI Help Tag", "VI Title", "VI Cust Title", "VI Help Use Url", "VI Help Url": Shortcut Menu Selection (User) {
            n163 = event-data() -> ("CtlRef"=w331:refnum<vi>, "ItemTag"=w329:string)  [unwired: 1 in]
            n164 = call "VIH Utility - APP - State Queue Parser (STR).vi"("input queue"=w329) -> ("state"=w328:string)  [unwired: 5 in, 3 out]
            n165 = case shown="\"Restore Value\"" w328 {
              tunnel: w331 -> [_ _ w337]
              tunnel: w330 -> [_ _ w339]
              frame Default {
              }
              frame "Select Help File" {
                n166 = call "File Dialog"("prompt"="Select a Help File", "pattern (all files)"="*.hlp;*.chm;*.htm;*.html;*.pdf") -> ("selected path"=w332:path, "error out"=w333:errorcluster)  [unwired: 10 in, 2 out]
                n167 = case shown="No Error" w333 {
                  tunnel: w332 -> [w336 _]
                  frame No Error {
                    n168 = property on="VI Help Path" class="Path"("Val(Sgnl)"=w336) -> ()  [unwired: 2 in, 2 out]
                  }
                  frame Error {
                  }
                }
              }
              frame "Restore Value" {
                n169 = Unbundle By Name(w339) -> ("VI Reference"=w338:refnum<vi>)
                n170 = property class="Ctl"(reference=w337) -> ("Label.Text"=w340:string)  [unwired: 1 in, 2 out]
                n171 = case shown="\"VI Help Url\"" w340 {
                  tunnel: w338 -> [_ w342 w345 w347 w350 w352 w356]
                  frame Default {
                    n172 = call <vilib>:"Beep.vi"() -> ()  [unwired: 12 in]
                  }
                  frame "VI Description" {
                    n173 = property class="VI"(reference=w342) -> ("Description"=w341:string)  [unwired: 1 in, 2 out]
                    n174 = property on="VI Description" class="Str"("Val(Sgnl)"=w341) -> ()  [unwired: 2 in, 2 out]
                  }
                  frame "VI Help Path" {
                    n175 = property class="VI"(reference=w345) -> ("Help.Path"=w344:path)  [unwired: 1 in, 2 out]
                    n176 = call "VIH - VI Doc Editor - Adjust Path.vi"("Path"=w344) -> ("Path out"=w343:path)  [unwired: 10 in]
                    n177 = property on="VI Help Path" class="Path"("Val(Sgnl)"=w343) -> ()  [unwired: 2 in, 2 out]
                  }
                  frame "VI Help Tag" {
                    n178 = property class="VI"(reference=w347) -> ("Help.Tag"=w346:string)  [unwired: 1 in, 2 out]
                    n179 = property on="VI Help Tag" class="Str"("Val(Sgnl)"=w346) -> ()  [unwired: 2 in, 2 out]
                  }
                  frame "VI Help Use Url" {
                    n180 = call "VIH Platform - LabVIEW - VI Property - Help - Use Web Url (2014).vi"("VI Refnum"=w350) -> ("UseWebURL out"=w349:bool)  [unwired: 8 in, 2 out]
                    n181 = Boolean To (0,1)(Boolean=w349) -> (0, 1=w348:i16)
                    n182 = property on="VI Help Use Url" class="Ring (strict)"("Val(Sgnl)"=w348) -> ()  [unwired: 2 in, 2 out]
                  }
                  frame "VI Help Url" {
                    n183 = call "VIH Platform - LabVIEW - VI Property - Help - Web Url (2014).vi"("VI Refnum"=w352) -> ("WebURL out"=w351:string)  [unwired: 8 in, 2 out]
                    n184 = property on="VI Help Url" class="Str"("Val(Sgnl)"=w351) -> ()  [unwired: 2 in, 2 out]
                  }
                  frame "VI Cust Title", "VI Title" {
                    n185 = property class="VI"(reference=w356) -> ("Front Panel.CustomTitle"=w355:bool, "Front Panel.Title"=w354:string)  [unwired: 1 in, 2 out]
                    n186 = Not(x=w355) -> (.not. x?=w353:bool)
                    n187 = property on="VI Cust Title" class="Bool (strict)"("Val(Sgnl)"=w353) -> ()  [unwired: 2 in, 2 out]
                    n188 = property on="VI Title" class="Str"("Val(Sgnl)"=w354) -> ()  [unwired: 2 in, 2 out]
                  }
                }
              }
            }
          }
          event "Ctrl Caption", "Ctrl Description", "Ctrl Tooltip": Value Change {
            n189 = event-data() -> ()  [unwired: 1 in, 1 out]
            n190 = Index Array(array=w360) -> (element=w359:string)  [unwired: 1 in]
            n191 = Format Into String(format string="Ctrl Props: Apply = %s;", w359) -> (resulting string=w358:string)  [unwired: 2 in, 1 out]
          }
          event "Ctrl Caption", "Ctrl Description", "Ctrl Tooltip": Shortcut Menu Activation? {
            n192 = event-data() -> ("MenuRef"=w361:refnum<k9>)  [unwired: 1 in, 1 out]
            n193 = call-poly "VIH Utility - MENU - Create Menu.vi"("Menu Description"="Re-read from VI   | Restore Value", "menu"=w361) -> ()  [unwired: 8 in, 2 out]
            n194 = event-data() -> ()  [unwired: 2 in, 1 out]
          }
          event "Ctrl Caption", "Ctrl Description", "Ctrl Tooltip": Shortcut Menu Selection (User) {
            n195 = event-data() -> ("CtlRef"=w368:refnum<vi>, "ItemTag"=w366:string)  [unwired: 1 in]
            n196 = call "VIH Utility - APP - State Queue Parser (STR).vi"("input queue"=w366) -> ("state"=w365:string)  [unwired: 5 in, 3 out]
            n197 = case shown="\"Restore Value\"" w365 {
              tunnel: w368 -> [_ w380]
              tunnel: w367 -> [_ _]
              tunnel: w364 -> [_ w375]
              tunnel: w363 -> [_ w374]
              frame Default {
              }
              frame "Restore Value" {
                n198 = for {
                  tunnel: w374 -> [w383] mode=indexing
                  tunnel: [w382] -> w376 mode=indexing
                  n199 = Unbundle By Name(w383) -> ("Tree Tag"=w382:string)
                }
                n200 = property class="Str"(reference=w380) -> ("Label.Text"=w381:string)  [unwired: 1 in, 2 out]
                n201 = Index Array(array=w375) -> (element=w377:string)  [unwired: 1 in]
                n202 = Search 1D Array(1D array=w376, element=w377) -> (index of element=w378:i32)  [unwired: 1 in]
                n203 = Index Array(array=w374, index=w378) -> (element=w379:T18)
                n204 = Unbundle By Name(w379) -> ("Page Refnum"=w369:refnum<vi>, "Ctl Refnum"=w372:refnum<vi>)
                n205 = Not A Number/Path/Refnum?(number/path/refnum=w372) -> (NaN/Path/Refnum?=w371:bool)
                n206 = Select(t=w369, s=w371, f=w372) -> (s? t:f=w370:refnum<vi>)
                n207 = call "VIH - VI Doc Editor #2 - GenObject Properties - Read.vi"("Gen Refnum"=w370) -> ("Props"=w373:T19)  [unwired: 7 in, 3 out]
                n208 = case shown="\"Ctrl Caption\"" w381 {
                  tunnel: w373 -> [_ w385 w387 w389]
                  frame Default {
                    n209 = call <vilib>:"Beep.vi"() -> ()  [unwired: 12 in]
                  }
                  frame "Ctrl Caption" {
                    n210 = Unbundle By Name(w385) -> ("Caption"=w384:string)
                    n211 = property on="Ctrl Caption" class="Str"("Val(Sgnl)"=w384) -> ()  [unwired: 2 in, 2 out]
                  }
                  frame "Ctrl Description" {
                    n212 = Unbundle By Name(w387) -> ("Description"=w386:string)
                    n213 = property on="Ctrl Description" class="Str"("Val(Sgnl)"=w386) -> ()  [unwired: 2 in, 2 out]
                  }
                  frame "Ctrl Tooltip" {
                    n214 = Unbundle By Name(w389) -> ("Tip Strip"=w388:string)
                    n215 = property on="Ctrl Tooltip" class="Str"("Val(Sgnl)"=w388) -> ()  [unwired: 2 in, 2 out]
                  }
                }
              }
            }
          }
          event "VI Icon": Mouse Down? {
            n216 = event-data() -> ()  [unwired: 1 in, 1 out]
            n217 = event-data("Button"=u16 2) -> ()  [unwired: 1 in, 1 out]
          }
          event "VI Icon": Shortcut Menu Activation? {
            (unwired) "Open VI Front Panel     | Open VI Front Panel\n--\nEdit VI Icon...         | VI Props: Edit Icon\nRe-read Icon from VI    | VI Props: Edit Icon = Restore"
            (unwired) "Open VI Front Panel     | Open VI Front Panel\nEdit VI Icon...         | VI Props: Edit Icon\n--\nRe-read icon from VI    | Restore Value\nRe-read VI Properties   | Restore VI Properties = VI"
            n218 = event-data() -> ("MenuRef"=w392:refnum<k9>)  [unwired: 1 in]
            n219 = call-poly "VIH Utility - MENU - Create Menu.vi"("Menu Description"="Edit VI Icon...         | VI Props: Edit Icon\n--\nRe-read Icon from VI    | VI Props: Edit Icon = Restore", "menu"=w392) -> ()  [unwired: 8 in, 2 out]
            n220 = event-data() -> ()  [unwired: 2 in, 1 out]
          }
          event "VI Icon": Shortcut Menu Selection (User) {
            n221 = event-data() -> ("ItemTag"=w394:string)  [unwired: 1 in, 2 out]
            n222 = call "VIH Utility - APP - State Queue Parser (STR).vi"("input queue"=w394) -> ("state"=w393:string)  [unwired: 5 in, 3 out]
            n223 = case shown="Default" w393 {
              tunnel: w394 -> [w399]
              tunnel: [w397] -> w395
              frame Default {
                n224 = Match Pattern(string=w399, regular expression=";$") -> (offset past match=w396:i32)  [unwired: 1 in, 3 out]
                n225 = case shown="..-1" w396 {
                  tunnel: w399 -> [w402 w403]
                  tunnel: [w401 w403] -> w397
                  frame ..-1 {
                    n226 = Concatenate Strings(w402, ";") -> (w401:string)
                  }
                  frame 0.. {
                  }
                }
              }
            }
          }
        }
      }
      frame "INIT" {
        (unwired) "EXIT;"
        n227 = call "VIH Utility - FILE - Get Path Attributes (Empty-NAP-Rel).vi"("Path"="VI Path in") -> ("Not A Path or Empty path"=w415:bool, "dup Path"=w414:path)  [unwired: 6 in, 3 out]
        n228 = property on="Conpane Image" class="Pict"("Erase First"=u8 0, "Origin"=T3 {"Horizontal"=0, "Vertical"=0}) -> ()  [unwired: 2 in, 2 out]
        n229 = case shown="True" w415 {
          selector: w415 -> [w431 _]
          tunnel: [w432 w436] -> w413
          tunnel: w414 -> [w432 _]
          tunnel: [w431 w438] -> w411
          tunnel: [_ w434] -> w412
          tunnel: [_ TRUE] -> w408
          frame False {
          }
          frame True {
            w435 = path ""  # Empty Path
            n230 = call <vilib>:"Menu Launch VI Information.vi"() -> ("Menu Launch:VI"=w443:string, "Menu Launch:App"=w434:refnum<vi>)  [unwired: 9 in, 1 out]
            n231 = Open VI Reference(application reference (local)=w434, vi path=w443) -> (vi reference=w445:refnum<vi>, error out=w444:errorcluster)  [unwired: 4 in]
            n232 = property class="VI" props=["Name", "Path"](reference=w445, error in=w444) -> (reference out=w447:refnum<vi>, error out=w446:errorcluster, "Path"=w437:path)  [unwired: 1 out]
            n233 = VI Library() -> (path=w441:path)
            n234 = Close Reference(reference=w447, error in (no error)=w446) -> ()  [unwired: 1 out]
            n235 = Strip Path(path=w441) -> (stripped path=w440:path)  [unwired: 1 out]
            n236 = call "VIH Utility - FILE - Get Path Attributes (Empty-NAP-Rel).vi"("Path"=w437) -> ("Not A Path or Empty path"=w442:bool, "dup Path"=w439:path)  [unwired: 6 in, 3 out]
            n237 = case shown="False" w442 {
              selector: w442 -> [w448 w458]
              tunnel: [w449 w458] -> w438
              tunnel: w440 -> [w454 _]
              tunnel: w439 -> [w450 _]
              frame False {
                n238 = call <vilib>:"Compare Two Paths.vi"("Path 2"=w450, "Path 1"=w454) -> ("Relative Path from 1 to 2"=w453:path)  [unwired: 6 in, 3 out]
                n239 = Path to Array of Strings(0:w453) -> (2:w452:string[])  [unwired: 1 out]
                n240 = Index Array(array=w452) -> (element=w451:string)  [unwired: 1 in]
                n241 = case shown="\"resource\"" w451 {
                  tunnel: [w455 TRUE TRUE] -> w449
                  tunnel: w448 -> [w455 _ _]
                  frame Default {
                  }
                  frame "project" {
                  }
                  frame "resource" {
                  }
                }
              }
              frame True {
              }
            }
            n242 = Select(t=w435, s=w438, f=w437) -> (s? t:f=w436:path)
          }
        }
        n243 = property on="Tab Control" class="TabCtl (strict)"("Value"=enum32{"VI Properties", "Control Properties"}."VI Properties" ("Tab Control")) -> ()  [unwired: 2 in, 2 out]
        n244 = property on="VI Help Use Url" class="Ring (strict)"("Visible"=w406) -> (error out=w405:errorcluster)  [unwired: 2 in, 1 out]
        n245 = call "VIH - VI Doc Editor #2 - GenObject Symbols.vi"("cmd (nop)"=T2."Init") -> ()  [unwired: 7 in, 4 out]
        n246 = property on="VI Help Url" class="Str"(error in=w405, "Visible"=FALSE) -> ()  [unwired: 1 in, 2 out]
        n247 = property on="%OpenVI" class="Bool"("Visible"=w408) -> ()  [unwired: 2 in, 2 out]
        n248 = Select(t="Ask For Select VI;\nUPDATE ALL;", s=w411, f="") -> (s? t:f=w417:string)
        n249 = Select(t=refnum<k0> refnum, s=w411, f=w412) -> (s? t:f=w409:refnum<vi>)
        n250 = local write "VI Path"(w413) -> ()
        n251 = local write "App Refnum"(w409) -> ()
        n252 = Concatenate Strings("UPDATE ALL;", w417, w430) -> (w427:string)
        "dup VI Path in" <- "VI Path in"
      }
      frame "UPDATE ALL" {
        n253 = Concatenate Strings("Set Busy = ON;\n\nClear Controls;\nSet Controls Size;\n\nOpen VI Reference;\nVI Props: Read From VI;\nVI Props: Changed?;\n\nUpdate VI Conpane Image;\n\nTree: Reset;\nTree: Message;\n\nDefer FP Update = ON;\n\nImage: Update;\n\nTree: Reset;\nTree: Build;\nTree: Preset Value;\nTree: Sort;\nTree: Disable Items;\nTree: Update Info = ALL;\n\nVI Props: Update;\nCtrl Props: Update;\nControl Appearance;\n\nKey Focus = Ctrl Tree;\n\nDefer FP Update = OFF;\nSet Busy = OFF;", w466) -> (w463:string)
      }
      frame "EXIT" {
        n254 = case shown="\"OK\"" w467 {
          tunnel: [_ TRUE] -> w475
          frame Default {
          }
          frame "OK" {
          }
        }
        "OK out" <- w475
        n255 = Format Into String(format string="Ask For Save VI = exit;\n\nClose VI Reference;\nClear Controls;\nTree: Reset;\nHALT = %s;", w467) -> (resulting string=w468:string)  [unwired: 2 in, 1 out]
      }
      frame "HALT" {
        # "to ensure VI Path is empty if the next call is made from the Tools menu"
        # "Force to close Front Panel if the VI resides in LV folder\n(the VI can be launched from the Tools menu; so it might run as top-level VI)"
        n256 = property class="VI"("Front Panel.Title"=w499) -> (error out=w488:errorcluster)  [unwired: 2 in, 1 out]
        n257 = control-ref of="Splitter 4"() -> (w498:refnum<vi>)
        n258 = Equal?(x=w485, y="CloseFP") -> (x = y?=w482:bool)
        n259 = property on="Property Node" class="Splitter"(reference=w498, "Locked"=FALSE ("Splitter Position Locked")) -> (error out=w489:errorcluster)  [unwired: 1 in, 1 out]
        n260 = property on="%OpenVI" class="Bool"("Visible"=TRUE) -> (error out=w486:errorcluster)  [unwired: 2 in, 1 out]
        n261 = local write "VI Path in"(path "") -> ()
        n262 = Merge Errors(w489, w488, w486) -> (w490:errorcluster)
        n263 = call <vilib>:"Clear Errors.vi"("error in (no error)"=w490) -> ("error out"=w491:errorcluster)  [unwired: 5 in, 1 out]
        n264 = VI Library() -> (path=w492:path)
        n265 = property class="VI"(error in=w491) -> ("Path"=w494:path)  [unwired: 1 in, 2 out]
        n266 = Strip Path(path=w492) -> (stripped path=w493:path)  [unwired: 1 out]
        n267 = call <vilib>:"Compare Two Paths.vi"("Path 2"=w494, "Path 1"=w493) -> ("Path 2 Relative to Path 1?"=w480:bool)  [unwired: 6 in, 3 out]
        n268 = Or(x=w482, y=w480) -> (x .or. y?=w483:bool)
        n269 = Not(x=w480) -> (.not. x?=w478:bool)
        n270 = And(x=w478, y=FALSE) -> (x .and. y?=w481:bool)
        n271 = case shown="True" w481 {
          frame False {
          }
          frame True {
            w506 = TRUE ("Visible")
            n272 = property on="VI Help Use Url" class="Ring (strict)"("Visible"=w506) -> ()  [unwired: 2 in, 2 out]
            n273 = property on="VI Help Url" class="Str"("Visible"=TRUE) -> ()  [unwired: 2 in, 2 out]
            n274 = property on="VI Help Path" class="Path"("Visible"=w506) -> ()  [unwired: 2 in, 2 out]
            n275 = property on="VI Help Tag" class="Str"("Visible"=w506) -> ()  [unwired: 2 in, 2 out]
          }
        }
        n276 = case shown="True" w483 {
          frame False {
          }
          frame True {
            n277 = invoke class="VI" method="FP.Close"() -> ()  [unwired: 3 in, 3 out]
          }
        }
      }
      frame "--------------------------------------- 1" {
      }
      frame "Set Busy" {
        n278 = case shown="\"ON\"" w518 {
          frame "OFF", Default {
            n279 = call <vilib>:"Unset Busy.vi"() -> ()  [unwired: 11 in, 1 out]
          }
          frame "ON" {
            n280 = call <vilib>:"Set Busy.vi"() -> ()  [unwired: 10 in, 2 out]
          }
        }
      }
      frame "Defer FP Update" {
        n281 = case shown="\"ON\"" w527 {
          tunnel: [_ TRUE] -> w525
          frame "OFF", Default {
          }
          frame "ON" {
          }
        }
        n282 = property class="VI"() -> ("Front Panel"=w526:refnum<vi>)  [unwired: 2 in, 2 out]
        n283 = property class="Pnl"(reference=w526, "Defer Panel Updates"=w525) -> ()  [unwired: 1 in, 2 out]
      }
      frame "Image: Update" {
        w531 = FALSE  # Shift
        w536 = FALSE
        n284 = Scan From String(format string="%d,%[^,],%[^,]", input string=w544, default 1=-1 ("default value 1"), default 2=w536, default 3=w536) -> (remaining string=w537:string, output 1=w541:i32, output 2=w535:bool)  [unwired: 3 in, 2 out]
        n285 = Unbundle By Name(w539) -> ("image"=w530:picture)
        n286 = case shown="0.." w541 {
          selector: w541 -> [_ w563]
          tunnel: w540 -> [_ w562]
          tunnel: w530 -> [w546 w561]
          tunnel: [w546 w559] -> w538
          tunnel: w537 -> [_ _]
          tunnel: w535 -> [_ w553]
          tunnel: w531 -> [_ w550]
          frame ..-1 {
          }
          frame 0.. {
            (unwired) u32 255 ("color(black)")
            (unwired) u32 16711680 ("color(black)")
            n287 = Index Array(array=w562, index=w563) -> (element=w560:T16)
            n288 = Unbundle By Name(w560) -> ("Bounds"=w558:cluster{"X0":i32, "Y0":i32, "X1":i32, "Y1":i32})
            n289 = Select(t=i16 2, s=w550, f=i16 1 ("Width")) -> (s? t:f=w547:i16)
            n290 = Bundle By Name(cluster=T4 {"Width"=1, "Style"=enum."Solid"} ("pen"), "Width"=w547) -> (w551:T4)
            n291 = in-place {
              n292 = in-place-cluster #1(w558) -> ("X0"=w572:i32, "Y0"=w567:i32, "X1"=w571:i32, "Y1"=w568:i32)
              n293 = Decrement(x=w567) -> (x-1=w566:i32)
              n294 = Increment(x=w568) -> (x+1=w565:i32)
              n295 = Decrement(x=w572) -> (x-1=w564:i32)
              n296 = Decrement(x=w564) -> (x-1=w570:i32)
              n297 = Increment(x=w571) -> (x+1=w569:i32)
              n298 = in-place-cluster #1("X0"=w570, "Y0"=w566, "X1"=w569, "Y1"=w565) -> (w557:cluster{"X0":i32, "Y0":i32, "X1":i32, "Y1":i32})
            }
            n299 = Select(t=u32 16711680 ("color(black)"), s=w553, f=u32 255 ("color(black)")) -> (s? t:f=w554:u32)
            n300 = call <vilib>:"Draw Rect.vi"("picture"=w561, "rect"=w557, "color(black)"=w554, "pen"=w551) -> ("new picture"=w559:picture)  [unwired: 5 in]
          }
        }
        "Conpane Image" <- w538
      }
      frame "Control Appearance" {
        n301 = Unbundle By Name(w580) -> ("VI Reference"=w576:refnum<vi>, "Changed"=w578:bool)
        n302 = Or Array Elements(Boolean array=w579) -> (logical OR=w577:bool)
        n303 = Or(x=w578, y=w577) -> (x .or. y?=w575:bool)
        n304 = case shown="True" w574 {
          tunnel: w583 -> [w588 w597]
          tunnel: [w588 w594] -> w582
          tunnel: w576 -> [_ w590]
          tunnel: w575 -> [_ w589]
          tunnel: [_ w589] -> w573
          frame False {
          }
          frame True {
            n305 = property class="VI"(reference=w590) -> ("Name"=w596:string)  [unwired: 1 in, 2 out]
            n306 = Select(t=" *", s=w589, f="") -> (s? t:f=w591:string)
            n307 = Format Into String(format string=" - %s%s", initial string=w597, w596, w591) -> (resulting string=w594:string)  [unwired: 1 in, 1 out]
          }
        }
        n308 = local write "Changed"(w573) -> ()
        n309 = call "VIH Utility - UI - Boolean to Control Disable Status.vi"("Status in"=w573) -> ("Control Disable if False"=w581:u8)  [unwired: 3 in, 1 out]
        n310 = property class="VI"("Front Panel.Title"=w582) -> ()  [unwired: 2 in, 2 out]
        n311 = property on="%Apply" class="Bool"("DisabledEnum"=w581) -> ()  [unwired: 2 in, 2 out]
        n312 = property on="%Apply&Save" class="Bool"("DisabledEnum"=w581) -> ()  [unwired: 2 in, 2 out]
      }
      frame "Clear Controls" {
        n313 = control-ref of="VI Version"() -> (w609:refnum<vi>)
        n314 = control-ref of="VI Cust Title"() -> (w610:refnum<vi>)
        n315 = control-ref of="VI Title"() -> (w611:refnum<vi>)
        n316 = control-ref of="VI Description"() -> (w612:refnum<vi>)
        n317 = control-ref of="VI Help Path"() -> (w613:refnum<vi>)
        n318 = control-ref of="VI Help Tag"() -> (w614:refnum<vi>)
        n319 = control-ref of="VI Help Use Url"() -> (w603:refnum<vi>)
        n320 = control-ref of="VI Help Url"() -> (w602:refnum<vi>)
        n321 = control-ref of="Ctrl Icon"() -> (w604:refnum<vi>)
        n322 = control-ref of="Ctrl Label"() -> (w615:refnum<vi>)
        n323 = control-ref of="Ctrl Caption"() -> (w619:refnum<vi>)
        n324 = control-ref of="Ctrl Description"() -> (w618:refnum<vi>)
        n325 = control-ref of="Ctrl Tooltip"() -> (w617:refnum<vi>)
        n326 = control-ref of="VI Icon"() -> (w608:refnum<vi>)
        n327 = Build Array(w608, w609, w610, w611, w612, w613, w614, w603, w602, w604, w615, w619, w618, w617) -> (w620:refnum<vi>[])
        n328 = for {
          tunnel: w620 -> [w626] mode=indexing
          n329 = invoke class="Ctl" method="Reinit To Default"(reference=w626) -> ()  [unwired: 2 in, 3 out]
        }
        n330 = call "VIH - VI Doc Editor #2 - GenObject Symbols.vi"("cmd (nop)"=T2."Init") -> ()  [unwired: 7 in, 4 out]
        n331 = property on="Ctrl Tree" class="Tree (strict)"("Value"=string[] [] ("Item Names")) -> ()  [unwired: 2 in, 2 out]
        n332 = property on="Ctrl Tree" class="Tree (strict)"("Active Item Tag"="TREE_COLUMN_HEADERS", "ActiveColNum"=-2 ("Active Cell:Active Column Number"), "CellFontBold"=FALSE ("Active Cell:Cell Font:Bold"), "CellFontColor"=u32 0) -> ()  [unwired: 2 in, 2 out]
        n333 = property on="Conpane Image" class="Pict"("Erase First"=u8 1) -> ()  [unwired: 2 in, 2 out]
      }
      frame "Key Focus" {
        n334 = case shown="\"Ctrl Tree\"" w631 {
          frame Default {
          }
          frame "Ctrl Tree" {
            n335 = property on="Ctrl Tree" class="Tree (strict)"("Key Focus"=TRUE) -> ()  [unwired: 2 in, 2 out]
          }
        }
      }
      frame "Set Controls Size" {
        w649 = 15 ("y")
        n336 = property on="Tab Control" class="TabCtl (strict)"() -> ("Left"=w658:i32, "Height"=w676:u32, "PaneWidth"=w655:u32)  [unwired: 2 in, 2 out]
        n337 = property on="VI Help Path" class="Path"() -> ("Height"=w670:u32)  [unwired: 2 in, 2 out]
        n338 = property on="VI Help Tag" class="Str"() -> ("Height"=w674:u32)  [unwired: 2 in, 2 out]
        n339 = To Long Integer(number=w655) -> (32bit integer=w639:i32)
        n340 = To Long Integer(number=w676) -> (32bit integer=w640:i32)
        n341 = To Long Integer(number=w674) -> (32bit integer=w638:i32)
        n342 = To Long Integer(number=w670) -> (32bit integer=w637:i32)
        n343 = Add(x=w649, y=w649) -> (x+y=w667:i32)
        n344 = Subtract(x=w639, y=w667) -> (x-y=w648:i32)
        n345 = Subtract(x=w640, y=15) -> (x-y=w673:i32)
        n346 = Subtract(x=w673, y=w638) -> (x-y=w660:i32)
        n347 = Add(x=w658, y=w649) -> (x+y=w657:i32)
        n348 = property on="Ctrl Icon" class="Pict"("Left"=w657) -> ("Width"=w656:u32)  [unwired: 2 in, 2 out]
        n349 = property on="VI Help Tag" class="Str"("Top"=w660, "Width"=w648) -> ()  [unwired: 2 in, 2 out]
        n350 = property on="Ctrl Tooltip" class="Str"("Top"=w660, "Width"=w648) -> ()  [unwired: 2 in, 2 out]
        n351 = Subtract(x=w660, y=3) -> (x-y=w672:i32)
        n352 = Subtract(x=w672, y=w637) -> (x-y=w651:i32)
        n353 = Add(x=w657, y=w656) -> (x+y=w653:u32)
        n354 = property on="Ctrl Description" class="Str"() -> ("Top"=w659:i32)  [unwired: 2 in, 2 out]
        n355 = Subtract(x=w639, y=w649) -> (x-y=w654:i32)
        n356 = property on="VI Help Path" class="Path"("Top"=w651, "Width"=w648) -> ()  [unwired: 2 in, 2 out]
        n357 = property on="VI Description" class="Str"() -> ("Top"=w644:i32)  [unwired: 2 in, 2 out]
        n358 = property on="VI Help Url" class="Str"("Top"=w651, "Width"=w648) -> ()  [unwired: 2 in, 2 out]
        n359 = Subtract(x=w654, y=w653) -> (x-y=w652:u32)
        n360 = property on="VI Help Use Url" class="Ring (strict)"() -> ("Width"=w646:u32)  [unwired: 2 in, 2 out]
        n361 = Subtract(x=w660, y=w659) -> (x-y=w663:i32)
        n362 = Subtract(x=w651, y=w644) -> (x-y=w665:i32)
        n363 = Subtract(x=w663, y=25) -> (x-y=w661:i32)
        n364 = To Long Integer(number=w646) -> (32bit integer=w635:i32)
        n365 = Subtract(x=w665, y=30) -> (x-y=w645:i32)
        n366 = property on="Ctrl Description" class="Str"("Height"=w661, "Width"=w648) -> ()  [unwired: 2 in, 2 out]
        n367 = Subtract(x=w648, y=w635) -> (x-y=w647:i32)
        n368 = property on="VI Description" class="Str"("Height"=w645, "Width"=w648) -> ()  [unwired: 2 in, 2 out]
        n369 = Add(x=w649, y=w647) -> (x+y=w650:i32)
        n370 = Add(x=w645, y=w644) -> (x+y=w643:i32)
        n371 = Add(x=w643, y=25) -> (x+y=w641:i32)
        n372 = property on="Ctrl Caption" class="Str"("Width"=w648) -> ()  [unwired: 2 in, 2 out]
        n373 = property on="VI Help Use Url" class="Ring (strict)"("Left"=w650, "Top"=w641) -> ()  [unwired: 2 in, 2 out]
        n374 = property on="VI Cust Title" class="Bool (strict)"() -> ("Width"=w669:u32)  [unwired: 2 in, 2 out]
        n375 = property on="VI Title" class="Str"("Width"=w648) -> ()  [unwired: 2 in, 2 out]
        n376 = To Long Integer(number=w669) -> (32bit integer=w636:i32)
        n377 = property on="Ctrl Label" class="Str"("Left"=w653, "Width"=w652) -> ()  [unwired: 2 in, 2 out]
        n378 = Subtract(x=w648, y=w636) -> (x-y=w664:i32)
        n379 = Add(x=w649, y=w664) -> (x+y=w668:i32)
        n380 = property on="VI Cust Title" class="Bool (strict)"("Left"=w668) -> ()  [unwired: 2 in, 2 out]
      }
      frame "Set Tab" {
        n381 = case shown="\"Ctl Props\"" w689 {
          tunnel: [enum32{"VI Properties", "Control Properties"}."VI Properties" ("y") enum32{"VI Properties", "Control Properties"}."Control Properties" ("y")] -> w687
          frame "VI Props", Default {
          }
          frame "Ctl Props" {
          }
        }
        n382 = Not Equal?(x=w687, y="Tab Control") -> (x != y?=w688:bool)
        n383 = case shown="True" w688 {
          tunnel: w687 -> [_ w696]
          tunnel: [_ "Defer FP Update = OFF;"] -> w683
          frame False {
          }
          frame True {
            n384 = property on="Tab Control" class="TabCtl (strict)"("Value"=w696) -> ()  [unwired: 2 in, 2 out]
          }
        }
        n385 = Concatenate Strings(w683, w685) -> (w684:string)
      }
      frame "--------------------------------------- 2" {
      }
      frame "Ask For Select VI" {
        n386 = local read "VI Path"() -> (w707:path)
        n387 = call "VIH Utility - FILE - Get Path Attributes (Empty-NAP-Rel).vi"("Path"=w707) -> ("Not A Path or Empty path"=w705:bool, "dup Path"=w706:path)  [unwired: 6 in, 3 out]
        n388 = case shown="False" w705 {
          tunnel: w706 -> [w723 _]
          tunnel: [w722 w724] -> w711
          frame False {
            n389 = Strip Path(path=w723) -> (stripped path=w722:path)  [unwired: 1 out]
          }
          frame True {
            w724 = path ""  # Not A Path
          }
        }
        n390 = call "File Dialog2"("start path"=w711, "prompt"="Select a VI", "pattern (all files)"="*.vi;*.vit") -> ("selected path"=w712:path, "error out"=w710:errorcluster)  [unwired: 9 in, 2 out]
        n391 = case shown="No Error" w710 {
          tunnel: w712 -> [w721 _]
          tunnel: w709 -> [w720 _]
          tunnel: [w720 _] -> w708
          frame No Error {
            n392 = local write "VI Path"(w721) -> ()
          }
          frame Error {
          }
        }
      }
      frame "Ask For Save VI" {
        n393 = case shown="True" "Changed" {
          tunnel: w732 -> [_ w741]
          tunnel: w731 -> [_ w744]
          tunnel: [T5."Continue" ("action") w739] -> w726
          frame False {
          }
          frame True {
            n394 = Empty String/Path?(string/path=w744) -> (empty?=w745:bool)
            n395 = Select(t="Continue", s=w745, f=w744) -> (s? t:f=w742:string)
            n396 = Format Into String(format string="\nYou have made changes that are not applied to the VI.\n\nWould you like to apply changes before %s?", w742) -> (resulting string=w740:string)  [unwired: 2 in, 1 out]
            n397 = call "VIH - VI Doc Editor - Dialog - Apply Changes.vi"("Title"=w741, "msg in"=w740) -> ("action"=w739:T5)  [unwired: 9 in]
          }
        }
        n398 = case shown="\"Continue\"" w726 {
          tunnel: [w748 w751 w753 "Defer FP Update = OFF;\nSet Busy = OFF;"] -> w730
          tunnel: w729 -> [w749 w752 w753 _]
          tunnel: "Apply to VI;" -> [w747 _ _ _]
          tunnel: "Apply to VI = SAVE;" -> [_ w750 _ _]
          frame "Apply" {
            n399 = Concatenate Strings(w747, w749) -> (w748:string)
          }
          frame "ApplySave" {
            n400 = Concatenate Strings(w750, w752) -> (w751:string)
          }
          frame "Continue" {
          }
          frame "Cancel" {
          }
        }
      }
      frame "--------------------------------------- 3" {
      }
      frame "Open VI Reference" {
        w776 = TRUE
        n401 = property class="App"() -> ("App.DefaultApplication"=w761:refnum<vi>)  [unwired: 2 in, 2 out]
        n402 = Not A Number/Path/Refnum?(number/path/refnum="App Refnum") -> (NaN/Path/Refnum?=w763:bool)
        n403 = Select(t=w761, s=w763, f="App Refnum") -> (s? t:f=w764:refnum<vi>)
        n404 = Open VI Reference(application reference (local)=w764, vi path="VI Path", options=3) -> (vi reference=w771:refnum<vi>, error out=w773:errorcluster)  [unwired: 3 in]
        n405 = Not(x=w773) -> (.not. x?=w772:bool)
        n406 = property class="VI"(reference=w771) -> (reference out=w770:refnum<vi>, "Name"=w769:string)  [unwired: 1 in, 1 out]
        n407 = local write "Good VI"(w772) -> ()
        n408 = Search and Replace String(replace all?=w776, case sensitive?=w776, input string=w769, search string="VI Helpeks.lvlib") -> (offset past replacement=w777:i32)  [unwired: 4 in, 3 out]
        n409 = Greater Or Equal To 0?(x=w777) -> (x >= 0?=w768:bool)
        n410 = case shown="True" w768 {
          tunnel: [w784 "Close VI Reference;\nClear Controls;\nTree: Reset;\n\nAsk For Select VI;\nUPDATE ALL;"] -> w767
          tunnel: w766 -> [w784 _]
          frame False {
          }
          frame True {
            w786 = path ""  # Empty Path
            n411 = local write "VI Path"(w786) -> ()
          }
        }
        n412 = Bundle By Name(cluster=T7 {"VI Reference"=refnum, "Changed"=FALSE, "Description"="", "Help.Path"=path "", "Help.Tag"="", "CustomTitle"=FALSE, "Title"="", "Icon"={"image type"=0, "image depth"=0, "image"=[], "mask"=[], "colors"=[], "Rectangle"={"left"=0, "top"=0, "right"=0, "bottom"=0}}, "Help.UseWebUrl"=FALSE, "Help.WebUrl"=""}, "VI Reference"=w770) -> (w780:T7)
      }
      frame "Close VI Reference" {
        n413 = property class="VI"("Front Panel.Title"=w797) -> ()  [unwired: 2 in, 2 out]
        n414 = for {
          tunnel: w796 -> [w803] mode=indexing
          tunnel: [w802] -> w795 mode=indexing
          tunnel: [w801] -> w789 mode=indexing
          n415 = Unbundle By Name(w803) -> ("Ctl Refnum"=w802:refnum<vi>, "Page Refnum"=w801:refnum<vi>)
        }
        n416 = Close Reference(reference=w795) -> (error out=w794:errorcluster)  [unwired: 1 in]
        n417 = Close Reference(reference=w789) -> (error out=w787:errorcluster)  [unwired: 1 in]
        n418 = local write "App Refnum"(refnum<k0> refnum) -> ()
        n419 = Merge Errors(w794, w787) -> (w788:errorcluster)
        n420 = Unbundle By Name(w793) -> ("VI Reference"=w792:refnum<vi>)
        n421 = Close Reference(reference=w792, error in (no error)=w788) -> ()  [unwired: 1 out]
      }
      frame "Open VI Front Panel" {
        n422 = Unbundle By Name(w804) -> ("VI Reference"=w805:refnum<vi>)
        n423 = property class="VI"(reference=w805) -> ("FP.Behavior"=w808:T9, "Exec.State"=w806:T8)  [unwired: 1 in, 2 out]
        n424 = Greater?(x=w806, y=T8."Idle" ("Execution:State")) -> (0:w811:bool)
        n425 = Equal?(x=T9."Modal" ("y"), y=w808) -> (x = y?=w810:bool)
        n426 = And(x=w810, y=w811) -> (x .and. y?=w813:bool)
        n427 = case shown="True" w813 {
          tunnel: [TRUE w822] -> w812
          tunnel: "The VI belongs to a running hierarchy and it's Front Panel is Modal.\n\nAre you sure to open the VI?" -> [_ w821]
          frame False {
          }
          frame True {
            n428 = Two Button Dialog(message=w821) -> (T button?=w822:bool)  [unwired: 2 in]
          }
        }
        n429 = case shown="True" w812 {
          tunnel: w805 -> [_ w823]
          frame False {
          }
          frame True {
            n430 = invoke class="VI" method="FP.Open"(reference=w823, "Activate"=TRUE ("Activate?")) -> ()  [unwired: 3 in, 5 out]
          }
        }
      }
      frame "Update VI Conpane Image" {
        n431 = Unbundle By Name(w841) -> ("VI Reference"=w840:refnum<vi>)
        n432 = case shown="True" w833 {
          tunnel: [w875 w883] -> w845
          tunnel: [_ w882] -> w844
          tunnel: [_ w881] -> w843
          tunnel: [_ w880] -> w842
          tunnel: w840 -> [w875 w879]
          tunnel: [_ w877] -> w831
          tunnel: [T10."Disabled and Grayed Out" ("Disabled") _] -> w832
          frame False {
          }
          frame True {
            n433 = property class="VI"(reference=w879) -> ("Path"=w878:path)  [unwired: 1 in, 2 out]
            n434 = call "VIH HelpGen - Get VI Conpane Image.vi"("Get Icon if no Conpane Image (F)"=TRUE, "Enable Check (T)"=TRUE, "VI Reference"=w879) -> ("error out"=w881:errorcluster, "Conpane Image"=w882:T6, "dup VI Reference"=w883:refnum<vi>)  [unwired: 6 in]
            n435 = invoke class="App" method="Get VI Editor Version"("VI Path"=w878) -> ("Get VI Editor Version"=w877:string)  [unwired: 4 in, 4 out]
            n436 = Strip Path(path=w878) -> (name=w880:string)  [unwired: 1 out]
          }
        }
        "VI Version" <- w831
        n437 = property on="VI Version" class="Str"("DisabledEnum"=w832) -> ()  [unwired: 2 in, 2 out]
        n438 = call "VIH Dialog - VI Terminals - Conpane Image.vi"("error in"=w843, "Conpane Image"=w844, "Original VI Name"=w842, "VI Reference"=w845) -> ("Rectangle"=w835:T20, "image"=w836:picture)  [unwired: 4 in, 2 out]
        n439 = property class="App"() -> ("App.Version"=w830:string)  [unwired: 2 in, 2 out]
        n440 = To Lower Case(string=w831) -> (all lower case string=w826:string)
        n441 = To Lower Case(string=w830) -> (all lower case string=w825:string)
        n442 = Unbundle By Name(w835) -> ("bottom"=w860:i16)
        n443 = property on="Conpane Image" class="Pict"() -> ("Bounds"=w856:T21, "Draw Area Size"=w855:T21)  [unwired: 2 in, 2 out]
        n444 = Bundle("image"=w836, "Rectangle"=w835) -> (w834:T22)  [unwired: 1 in]
        n445 = Not Equal?(x=w825, y=w826) -> (x != y?=w829:bool)
        n446 = To Long Integer(number=w860) -> (32bit integer=w847:i32)
        n447 = case shown="True" w829 {
          selector: w829 -> [_ w873]
          tunnel: [_ w873] -> w828
          tunnel: [u32 16777222 w865] -> w827
          tunnel: w826 -> [_ w872]
          tunnel: w825 -> [_ w871]
          frame False {
          }
          frame True {
            n448 = Fract/Exp String To Number(use system decimal point (T)=FALSE, string=w871) -> (number=w867:dbl)  [unwired: 2 in, 1 out]
            n449 = Fract/Exp String To Number(use system decimal point (T)=FALSE, string=w872) -> (number=w868:dbl)  [unwired: 2 in, 1 out]
            n450 = Not Equal?(x=w867, y=w868) -> (x != y?=w866:bool)
            n451 = Select(t=u32 16711680, s=w866, f=u32 16777222) -> (s? t:f=w865:u32)
          }
        }
        n452 = Unbundle By Name(w856) -> ("Height"=w851:u32)
        n453 = Unbundle By Name(w855) -> ("Height"=w850:u32)
        n454 = Add(x=w847, y=5) -> (x+y=w852:i32)
        n455 = To Long Integer(number=w851) -> (32bit integer=w854:i32)
        n456 = To Long Integer(number=w850) -> (32bit integer=w853:i32)
        n457 = Subtract(x=w854, y=w853) -> (x-y=w849:i32)
        n458 = Add(x=w852, y=w849) -> (x+y=w848:i32)
        n459 = control-ref of="Splitter 4"() -> (w846:refnum<vi>)
        n460 = Max & Min(x=50 ("Splitter Position"), y=w848) -> (max(x,y)=w857:i32)  [unwired: 1 out]
        n461 = property on="VI Version" class="Str"("Text.FontBold"=w828, "Text.FontColor"=w827) -> ()  [unwired: 2 in, 2 out]
        n462 = stacked-sequence {
          tunnel: w857 -> [w886]
          tunnel: w846 -> [w885]
          frame #0 {
            n463 = property on="Property Node" class="Splitter"(reference=w885, "Locked"=FALSE ("Splitter Position Locked"), "Position"=w886, "Locked"=TRUE ("Splitter Position Locked")) -> ()  [unwired: 1 in, 2 out]
          }
        }
      }
      frame "--------------------------------------- 4" {
      }
      frame "Tree: Build" {
        n464 = Unbundle By Name(w924) -> ("VI Reference"=w906:refnum<vi>)
        n465 = control-ref of="Ctrl Tree"() -> (w915:refnum<vi>)
        n466 = Unbundle(w909) -> ("image"=w908:picture, "Rectangle"=w907:T20)
        n467 = for {
          tunnel: w895 -> [w954] mode=indexing
          shift-right: [w950] -> w905
          shift-left: w915 -> [w955]
          tunnel: [w949] -> w904 mode=indexing
          n468 = invoke class="Tree (strict)" method="Edit Tree Items.Add Item to End"(reference=w955, "Left Cell"=w954) -> (reference out=w953:refnum<vi>, "Edit Tree Items:Add Item to End"=w949:string)  [unwired: 6 in, 6 out]
          n469 = property class="Tree (strict)"(reference=w953, "Active Item Tag"=w949, "ActiveColNum"=-2 ("Active Cell:Active Column Number"), "CellFontBold"=TRUE ("Active Cell:Cell Font:Bold"), "CellBG"=u32 16777152) -> (reference out=w950:refnum<vi>)  [unwired: 1 in, 1 out]
        }
        n470 = Unbundle(w907) -> ("left"=w927:i16, "top"=w928:i16)  [unwired: 2 out]
        n471 = call <vilib>:"Picture to Pixmap.vi"("depth"=24, "picture"=w908) -> ("image data"=w932:T6)  [unwired: 8 in, 1 out]
        n472 = Bundle("top"=w928, "left"=w927) -> (w926:cluster{"top":i16, "left":i16})  [unwired: 1 in]
        n473 = call "VIH HelpGen - Get VI Conpane Control Refnums.vi"("Sort terminals (T)"=TRUE, "VI Reference"=w906) -> ("error out"=w933:errorcluster, "Ctrl Attributes"=w925:T23[], "Conpane Ctrl Refnums"=w930:refnum<vi>[], "dup VI Reference"=w923:refnum<vi>)  [unwired: 6 in]
        n474 = call "VIH HelpGen - Image - Find Ctrl Area in Conpane Picture.vi"("Conpane Image Data"=w932, "error in"=w933, "Top Left"=w926, "Ctrl Attributes"=w925, "Conpane Ctrl Refnums"=w930) -> ("error out"=w934:errorcluster, "Terminals Info"=w917:T15, "dup Conpane Ctrl Refnums"=w929:refnum<vi>[])  [unwired: 2 in, 2 out]
        n475 = Index Array(array=w904) -> (element #1=w914:string, element #2=w913:string)  [unwired: 2 in]
        n476 = call "VIH - VI Doc Editor #2 - Build Control Tree.vi"("Ctrl Attributes"=w925, "Expand Tab Control (F)"=TRUE, "error in"=w934, "Parent tag"=w914, "Tree Refnum"=w905, "Ctrl Refnums"=w929) -> ("error out"=w920:errorcluster, "Controls Info"=w903:T18[], "dup Ctrl Refnums"=w922:refnum<vi>[])  [unwired: 3 in]
        n477 = call "VIH - VI Doc Editor #2 - Get Non-terminal GenObject Refnums.vi"("error in"=w920, "Conpane Ctrl Refnums"=w922, "VI Reference"=w923) -> ("error out"=w919:errorcluster, "Non-terminal GenObject Refnums"=w921:refnum<vi>[])  [unwired: 6 in, 1 out]
        n478 = call "VIH - VI Doc Editor #2 - Build Control Tree.vi"("Expand Tab Control (F)"=TRUE, "error in"=w919, "Parent tag"=w913, "Tree Refnum"=w905, "Ctrl Refnums"=w921) -> ("Controls Info"=w902:T18[])  [unwired: 4 in, 2 out]
        n479 = Empty Array?(array=w903) -> (empty?=w901:bool)
        n480 = Empty Array?(array=w902) -> (empty?=w900:bool)
        n481 = Build Array (concatenate)(w903, w902) -> (w918:T18[])
        n482 = Build Array(w901, w900) -> (w899:bool[])
        n483 = for {
          tunnel: w905 -> [w940]
          tunnel: w904 -> [w939] mode=indexing
          tunnel: w899 -> [w938] mode=indexing
          tunnel: "<none>" -> [w937]
          n484 = case shown="True" w938 {
            tunnel: w940 -> [_ w947]
            tunnel: w939 -> [_ w946]
            tunnel: w937 -> [_ w945]
            frame False {
            }
            frame True {
              n485 = invoke class="Tree (strict)" method="Edit Tree Items.Add Item"(reference=w947, "Parent Tag"=w946, "Left Cell"=w945) -> (reference out=w944:refnum<vi>, error out=w943:errorcluster, "Edit Tree Items:Add Item"=w942:string)  [unwired: 6 in, 6 out]
              n486 = property class="Tree (strict)"(reference=w944, error in=w943, "Active Item Tag"=w942, "Disabled?"=TRUE) -> ()  [unwired: 2 out]
            }
          }
        }
        n487 = Array Size(array=w918) -> (size(s)=w912:i32)
        n488 = Reshape Array(w917, w912) -> (w916:T15)
        n489 = Initialize Array(FALSE, w912) -> (w910:bool[])
      }
      frame "Tree: Preset Value" {
        n490 = property on="Ctrl Tree" class="Tree (strict)"("Value"=string[] [] ("Ctrl Tree")) -> (error out=w956:errorcluster)  [unwired: 2 in, 1 out]
        n491 = call "VIH - VI Doc Editor #2 - GenObject Symbols.vi"("cmd (nop)"=T2."get symbols") -> ("Symbols"=w963:T6[])  [unwired: 7 in, 3 out]
        n492 = invoke on="Ctrl Tree" class="Tree (strict)" method="Custom Item Symbols.Set Symbol Array"(error in=w956, "glyphs"=w963) -> (error out=w959:errorcluster)  [unwired: 2 in, 3 out]
        n493 = call <vilib>:"Clear Errors.vi"("error in (no error)"=w959) -> ("error out"=w958:errorcluster)  [unwired: 5 in, 1 out]
        n494 = invoke on="Ctrl Tree" class="Tree (strict)" method="Open/Close.Open/Close All"(error in=w958, "Open"=FALSE ("Open?")) -> (error out=w957:errorcluster)  [unwired: 2 in, 3 out]
        n495 = for {
          tunnel: w957 -> [w972]
          tunnel: w960 -> [w971] mode=indexing
          n496 = invoke on="Ctrl Tree" class="Tree (strict)" method="Open/Close.Item"(error in=w972, "tag"=w971, "Open"=TRUE ("Open?")) -> ()  [unwired: 2 in, 5 out]
        }
      }
      frame "Tree: Sort" {
        w987 = "TREE_COLUMN_HEADERS"
        n497 = To Upper Case(1:w982) -> (0:w981:string)
        n498 = Equal?(x=w981, y="MODE1") -> (x = y?=w974:bool)
        n499 = Unbundle By Name("Sort") -> ("Column"=w985:i32, "Reverse"=w986:bool)
        n500 = case shown="True" w974 {
          tunnel: w976 -> [w998 w1001]
          tunnel: [w998 w1000] -> w975
          frame False {
          }
          frame True {
            n501 = Array Subset(array=w1001, index=1) -> (w1000:string[])  [unwired: 1 in]
          }
        }
        n502 = for {
          tunnel: w975 -> [w1013] mode=indexing
          tunnel: w986 -> [w1012]
          tunnel: w985 -> [w1011]
          tunnel: [w1010] -> w977
          n503 = invoke on="Ctrl Tree" class="Tree (strict)" method="Edit Tree Items.Sort Children"("tag"=w1013, "Sort Column"=w1011, "Case Sensitivity"=2, "Sort Recursively"=TRUE ("Sort Recursively?"), "Reverse Order"=w1012) -> (error out=w1010:errorcluster)  [unwired: 3 in, 7 out]
        }
        n504 = property on="Ctrl Tree" class="Tree (strict)"(error in=w977, "Active Item Tag"=w987, "ActiveColNum"=-2 ("Active Cell:Active Column Number"), "CellFontBold"=FALSE ("Active Cell:Cell Font:Bold"), "CellFontColor"=u32 0) -> (error out=w978:errorcluster)  [unwired: 1 in, 1 out]
        n505 = Not(x=w974) -> (.not. x?=w979:bool)
        n506 = Greater Or Equal To 0?(x=w985) -> (x >= 0?=w984:bool)
        n507 = And(x=w979, y=w984) -> (x .and. y?=w983:bool)
        n508 = case shown="True" w983 {
          tunnel: w987 -> [_ w1008]
          tunnel: w986 -> [_ w1004]
          tunnel: w985 -> [_ w1003]
          tunnel: w978 -> [_ w1002]
          frame False {
          }
          frame True {
            n509 = Select(t=u32 16860, s=w1004, f=u32 0) -> (s? t:f=w1006:u32)
            n510 = property on="Ctrl Tree" class="Tree (strict)"(error in=w1002, "Active Item Tag"=w1008, "ActiveColNum"=w1003, "CellFontBold"=TRUE ("Active Cell:Cell Font:Bold"), "CellFontColor"=w1006) -> ()  [unwired: 1 in, 2 out]
          }
        }
      }
      frame "Tree: Disable Items" {
      }
      frame "Tree: Reset" {
        n511 = invoke on="Ctrl Tree" class="Tree (strict)" method="Edit Tree Items.Delete"() -> (error out=w1027:errorcluster)  [unwired: 5 in, 4 out]
        n512 = invoke on="Ctrl Tree" class="Tree (strict)" method="Custom Item Symbols.Revert Symbols"(error in=w1027) -> ()  [unwired: 2 in, 3 out]
      }
      frame "Tree: Message" {
        n513 = invoke on="Ctrl Tree" class="Tree (strict)" method="Edit Tree Items.Add Item to End"("Left Cell"="Collecting information..." ("Left Cell String")) -> ()  [unwired: 7 in, 8 out]
      }
      frame "Tree: Open Items" {
        n514 = for {
          tunnel: w1039 -> [w1044] mode=indexing
          n515 = invoke on="Ctrl Tree" class="Tree (strict)" method="Open/Close.Item"("tag"=w1044, "Open"=TRUE) -> ()  [unwired: 3 in, 5 out]
        }
      }
      frame "Tree: Update Info" {
        n516 = for {
          tunnel: w1050 -> [w1061] mode=indexing
          tunnel: [w1060] -> w1051 mode=indexing
          n517 = Unbundle By Name(w1061) -> ("Tree Tag"=w1060:string)
        }
        n518 = case shown="\"ALL\"" w1047 {
          selector: w1047 -> [_ _ w1059]
          tunnel: [w1056 w1057 w1058] -> w1046
          tunnel: w1045 -> [w1056 _ _]
          frame "" {
          }
          frame "ALL" {
            n519 = property on="Ctrl Tree" class="Tree (strict)"() -> ("All Tags"=w1057:string[])  [unwired: 2 in, 2 out]
          }
          frame Default {
            n520 = Build Array(w1059) -> (w1058:string[])
          }
        }
        n521 = for {
          tunnel: w1051 -> [w1067]
          tunnel: w1050 -> [w1066]
          tunnel: w1046 -> [w1065] mode=indexing
          shift-right: [w1062] -> w1048
          shift-left: w1049 -> [w1063]
          n522 = Search 1D Array(1D array=w1067, element=w1065) -> (index of element=w1064:i32)  [unwired: 1 in]
          n523 = case shown="0.." w1064 {
            selector: w1064 -> [_ w1079]
            tunnel: w1066 -> [_ w1089]
            tunnel: w1065 -> [_ w1083]
            tunnel: w1063 -> [w1068 w1081]
            tunnel: [w1068 w1080] -> w1062
            frame ..-1 {
            }
            frame 0.. {
              n524 = Index Array(array=w1089, index=w1079) -> (element=w1088:T18)
              n525 = Unbundle By Name(w1088) -> ("Ctl Caption"=w1087:string, "Ctl Description"=w1086:string, "Ctl Tooltip"=w1085:string, "Page Refnum"=w1070:refnum<vi>, "Ctl Refnum"=w1071:refnum<vi>)
              n526 = Not A Number/Path/Refnum?(number/path/refnum=w1071) -> (NaN/Path/Refnum?=w1072:bool)
              n527 = Build Array(w1087, w1086, w1085) -> (w1084:string[])
              n528 = Select(t=w1070, s=w1072, f=w1071) -> (s? t:f=w1069:refnum<vi>)
              n529 = call "VIH - VI Doc Editor #2 - GenObject Properties - Read.vi"("Gen Refnum"=w1069) -> ("Props"=w1076:T19)  [unwired: 7 in, 3 out]
              n530 = Unbundle(w1076) -> ("Caption"=w1075:string, "Description"=w1074:string, "Tip Strip"=w1073:string)  [unwired: 1 out]
              n531 = Build Array(w1075, w1074, w1073) -> (w1077:string[])
              n532 = for {
                tunnel: w1084 -> [w1091] mode=indexing
                tunnel: w1083 -> [w1102]
                tunnel: [w1094] -> w1082 mode=indexing
                tunnel: w1077 -> [w1092] mode=indexing
                i -> [w1101]
                n533 = Empty String/Path?(string/path=w1092) -> (empty?=w1098:bool)
                n534 = Not Equal?(x=w1091, y=w1092) -> (x != y?=w1094:bool)
                n535 = Select(t="-", s=w1098, f="+") -> (s? t:f=w1093:string)
                n536 = Add(x=w1101, y=2) -> (x+y=w1100:i32)
                n537 = Select(t="new", s=w1094, f=w1093) -> (s? t:f=w1095:string)
                n538 = property on="Ctrl Tree" class="Tree (strict)"("Active Item Tag"=w1102, "ActiveColNum"=w1100, "Cell String"=w1095) -> ()  [unwired: 2 in, 2 out]
              }
              n539 = Or Array Elements(Boolean array=w1082) -> (logical OR=w1078:bool)
              n540 = Replace Array Subset(array=w1081, new element=w1078, index=w1079) -> (w1080:bool[])
            }
          }
        }
      }
      frame "--------------------------------------- 5" {
      }
      frame "VI Props: Read From VI" {
        n541 = Unbundle By Name(w1111) -> ("VI Reference"=w1109:refnum<vi>)
        n542 = in-place {
          in-place-border: w1109 -> [w1124]
          w1131 = FALSE  # Changed
          n543 = in-place-cluster #2(w1111) -> ()  [unwired: 9 out]
          n544 = property class="VI"(reference=w1124) -> (reference out=w1117:refnum<vi>, "Description"=w1126:string, "Help.Path"=w1121:path, "Help.Tag"=w1127:string, "Front Panel.CustomTitle"=w1128:bool, "Front Panel.Title"=w1129:string)  [unwired: 1 in, 1 out]
          n545 = invoke class="VI" method="VI Icon.Get as Image Data"(reference=w1117) -> (reference out=w1118:refnum<vi>, error out=w1125:errorcluster, "ImageData"=w1132:T6)  [unwired: 5 in, 3 out]
          n546 = call "VIH - VI Doc Editor - Adjust Path.vi"("Path"=w1121) -> ("Path out"=w1120:path)  [unwired: 10 in]
          n547 = case shown="No Error" w1125 {
            tunnel: w1132 -> [w1133 _]
            tunnel: [w1133 _] -> w1130
            frame No Error {
            }
            frame Error {
            }
          }
          n548 = call "VIH Platform - LabVIEW - VI Property - Help - Use Web Url (2014).vi"("VI Refnum"=w1118) -> ("UseWebURL out"=w1123:bool, "dup VI Refnum"=w1119:refnum<vi>)  [unwired: 8 in, 1 out]
          n549 = call "VIH Platform - LabVIEW - VI Property - Help - Web Url (2014).vi"("VI Refnum"=w1119) -> ("WebURL out"=w1122:string)  [unwired: 8 in, 2 out]
          n550 = in-place-cluster #2("Changed"=w1131, "Description"=w1126, "Help.Path"=w1120, "Help.Tag"=w1127, "CustomTitle"=w1128, "Title"=w1129, "Icon"=w1130, "Help.UseWebUrl"=w1123, "Help.WebUrl"=w1122) -> (w1110:T7)
        }
      }
      frame "VI Props: Changed?" {
        n551 = Unbundle By Name(w1156) -> ("VI Reference"=w1146:refnum<vi>, "Description"=w1155:string, "Help.Path"=w1154:path, "Help.Tag"=w1153:string, "CustomTitle"=w1152:bool, "Title"=w1151:string, "Icon"=w1139:T6, "Help.UseWebUrl"=w1148:bool, "Help.WebUrl"=w1147:string)
        n552 = property class="VI"(reference=w1146) -> (reference out=w1135:refnum<vi>, "Description"=w1163:string, "Help.Path"=w1138:path, "Help.Tag"=w1162:string, "Front Panel.CustomTitle"=w1161:bool, "Front Panel.Title"=w1160:string)  [unwired: 1 in, 1 out]
        n553 = invoke class="VI" method="VI Icon.Get as Image Data"(reference=w1135) -> (reference out=w1134:refnum<vi>, "ImageData"=w1140:T6)  [unwired: 5 in, 4 out]
        n554 = call "VIH - VI Doc Editor - Adjust Path.vi"("Path"=w1138) -> ("Path out"=w1137:path)  [unwired: 10 in]
        n555 = call "VIH Platform - LabVIEW - VI Property - Help - Use Web Url (2014).vi"("VI Refnum"=w1134) -> ("UseWebURL out"=w1145:bool, "dup VI Refnum"=w1136:refnum<vi>)  [unwired: 8 in, 1 out]
        n556 = Bundle("Description"=w1155, "Help.Path"=w1154, "Help.Tag"=w1153, "CustomTitle"=w1152, "Title"=w1151, "Help.UseWebUrl"=w1148, "Help.WebUrl"=w1147) -> (w1149:T24)  [unwired: 1 in]
        n557 = call "VIH Platform - LabVIEW - VI Property - Help - Web Url (2014).vi"("VI Refnum"=w1136) -> ("WebURL out"=w1144:string)  [unwired: 8 in, 2 out]
        n558 = Not Equal?(x=w1140, y=w1139) -> (x != y?=w1142:bool)
        n559 = Bundle(cluster=w1149, "Description"=w1163, "Help.Path"=w1137, "Help.Tag"=w1162, "CustomTitle"=w1161, "Title"=w1160, "Help.UseWebUrl"=w1145, "Help.WebUrl"=w1144) -> (w1150:T24)
        n560 = Not Equal?(x=w1150, y=w1149) -> (x != y?=w1143:bool)
        n561 = Or(x=w1143, y=w1142) -> (x .or. y?=w1141:bool)
        n562 = Bundle By Name(cluster=w1156, "Changed"=w1141) -> (w1157:T7)
      }
      frame "VI Props: Update" {
        n563 = case shown="True" w1173 {
          tunnel: w1184 -> [_ w1199]
          tunnel: [_ w1198] -> w1183
          tunnel: [_ w1197] -> w1182
          tunnel: [_ w1190] -> w1180
          tunnel: [_ w1194] -> w1178
          tunnel: [_ w1196] -> w1176
          tunnel: [_ w1195] -> w1175
          tunnel: [_ w1194] -> w1174
          tunnel: [T10."Disabled and Grayed Out" ("Disabled") _] -> w1170
          tunnel: [_ w1193] -> w1168
          tunnel: [_ w1192] -> w1171
          frame False {
          }
          frame True {
            n564 = Unbundle By Name(w1199) -> ("Description"=w1198:string, "Help.Path"=w1195:path, "Help.Tag"=w1197:string, "CustomTitle"=w1194:bool, "Title"=w1196:string, "Icon"=w1191:T6, "Help.UseWebUrl"=w1193:bool, "Help.WebUrl"=w1192:string)  [unwired: 2 out]
            n565 = call <vilib>:"Draw Flattened Pixmap.vi"("image data"=w1191) -> ("new picture"=w1190:picture)  [unwired: 8 in]
          }
        }
        "VI Icon" <- w1180
        n566 = Not(x=w1178) -> (.not. x?=w1179:bool)
        n567 = call "VIH Utility - UI - Boolean to Control Disable Status.vi"("Status in"=w1174) -> ("Control Disable if False"=w1177:u8)  [unwired: 3 in, 1 out]
        n568 = property on="VI Description" class="Str"("Value"=w1183, "DisabledEnum"=w1170) -> ()  [unwired: 2 in, 2 out]
        n569 = property on="VI Title Default" class="Bool (strict)"("Value"=w1179, "DisabledEnum"=w1170) -> ()  [unwired: 2 in, 2 out]
        n570 = property on="VI Title" class="Str"("DisabledEnum"=w1177, "Value"=w1176) -> ()  [unwired: 2 in, 2 out]
        n571 = property on="VI Icon" class="Pict"("DisabledEnum"=w1170) -> ()  [unwired: 2 in, 2 out]
        n572 = Not(x=w1168) -> (.not. x?=w1169:bool)
        n573 = Boolean To (0,1)(Boolean=w1168) -> (0, 1=w1172:i16)
        n574 = property on="VI Help Path" class="Path"("Value"=w1175, "DisabledEnum"=w1170, "Visible"=w1169) -> ()  [unwired: 2 in, 2 out]
        n575 = property on="VI Help Tag" class="Str"("Value"=w1182, "DisabledEnum"=w1170, "Visible"=w1169) -> ()  [unwired: 2 in, 2 out]
        n576 = property on="VI Help Url" class="Str"("Value"=w1171, "DisabledEnum"=w1170, "Visible"=w1168) -> ()  [unwired: 2 in, 2 out]
        n577 = property on="VI Help Use Url" class="Ring (strict)"("Value"=w1172, "DisabledEnum"=w1170, "Visible"=w1167) -> ()  [unwired: 2 in, 2 out]
      }
      frame "VI Props: Apply" {
        n578 = in-place {
          n579 = in-place-cluster #3(w1204) -> ()  [unwired: 7 out]
          n580 = Greater Than 0?(x="VI Help Use Url") -> (x > 0?=w1212:bool)
          n581 = call "VIH - VI Doc Editor - Adjust Path.vi"("Path"="VI Help Path") -> ("Path out"=w1209:path)  [unwired: 10 in]
          n582 = Not(x="VI Cust Title") -> (.not. x?=w1214:bool)
          n583 = in-place-cluster #3("Description"="VI Description", "Help.Path"=w1209, "Help.Tag"="VI Help Tag", "CustomTitle"=w1214, "Title"="VI Title", "Help.UseWebUrl"=w1212, "Help.WebUrl"="VI Help Url") -> (w1203:T7)
        }
        n584 = Concatenate Strings("Defer FP Update = ON;\n\nVI Props: Update;\nVI Props: Changed?;\n\nControl Appearance;\n\nDefer FP Update = OFF;", w1208) -> (w1202:string)
      }
      frame "VI Props: Edit Icon" {
        n585 = Unbundle By Name(w1220) -> ("VI Reference"=w1219:refnum<vi>)
        n586 = in-place {
          in-place-border: w1221 -> [w1232]
          in-place-border: w1219 -> [w1231]
          n587 = in-place-cluster #4(w1220) -> ("Icon"=w1233:T6)
          n588 = case shown="Default" w1232 {
            tunnel: [w1238 w1243] -> w1234
            tunnel: w1233 -> [w1236 _]
            tunnel: w1231 -> [_ w1244]
            tunnel: [FALSE _] -> w1230
            frame Default {
              n589 = invoke class="App" method="UI.Edit Icon"("Color 256"=w1236) -> (error out=w1239:errorcluster, "Color 256"=w1240:T6)  [unwired: 8 in, 7 out]
              n590 = case shown="No Error" w1239 {
                tunnel: w1240 -> [w1241 _]
                tunnel: [w1241 w1242] -> w1238
                tunnel: w1236 -> [_ w1242]
                frame No Error {
                }
                frame Error {
                }
              }
            }
            frame "Restore" {
              n591 = invoke class="VI" method="VI Icon.Get as Image Data"(reference=w1244) -> ("ImageData"=w1243:T6)  [unwired: 5 in, 5 out]
            }
          }
          n592 = case shown="True" w1230 {
            frame False {
            }
            frame True {
              n593 = Wait (ms)(milliseconds to wait=u32 50) -> ()  [unwired: 1 out]
            }
          }
          n594 = in-place-cluster #4("Icon"=w1234) -> (w1223:T7)
        }
        n595 = Concatenate Strings("Defer FP Update = ON;\n\nVI Props: Update;\nVI Props: Changed?;\n\nControl Appearance;\n\nDefer FP Update = OFF;", w1229) -> (w1225:string)
      }
      frame "--------------------------------------- 6" {
      }
      frame "Ctrl Props: Read From VI" {
        n596 = for {
          tunnel: w1255 -> [w1289] mode=indexing
          tunnel: [w1288] -> w1254 mode=indexing
          n597 = Unbundle By Name(w1289) -> ("Tree Tag"=w1288:string)
        }
        n598 = case shown="\"ALL\"" w1258 {
          selector: w1258 -> [_ _ w1293]
          tunnel: [w1290 w1291 w1292] -> w1256
          tunnel: w1257 -> [w1290 _ _]
          frame "" {
          }
          frame "ALL" {
            n599 = property on="Ctrl Tree" class="Tree (strict)"() -> ("All Tags"=w1291:string[])  [unwired: 2 in, 2 out]
          }
          frame Default {
            n600 = Build Array(w1293) -> (w1292:string[])
          }
        }
        n601 = for {
          tunnel: w1254 -> [w1269]
          tunnel: w1256 -> [w1267] mode=indexing
          shift-right: [w1264] -> w1252
          shift-left: w1253 -> [w1265]
          shift-right: [w1263] -> w1251
          shift-left: w1255 -> [w1268]
          n602 = Search 1D Array(1D array=w1269, element=w1267) -> (index of element=w1266:i32)  [unwired: 1 in]
          n603 = case shown="0.." w1266 {
            selector: w1266 -> [_ w1274]
            tunnel: w1268 -> [w1270 w1275]
            tunnel: w1265 -> [w1271 w1276]
            tunnel: [w1271 w1273] -> w1264
            tunnel: [w1270 w1272] -> w1263
            frame ..-1 {
            }
            frame 0.. {
              n604 = in-place {
                n605 = in-place-array #5(w1275, w1274) -> (w1277:T18)
                n606 = in-place-array #6(w1276, w1274) -> ()  [unwired: 1 out]
                n607 = Unbundle By Name(w1277) -> ("Page Refnum"=w1279:refnum<vi>, "Ctl Refnum"=w1281:refnum<vi>)
                n608 = Not A Number/Path/Refnum?(number/path/refnum=w1281) -> (NaN/Path/Refnum?=w1280:bool)
                n609 = Select(t=w1279, s=w1280, f=w1281) -> (s? t:f=w1278:refnum<vi>)
                n610 = call "VIH - VI Doc Editor #2 - GenObject Properties - Read.vi"("Gen Refnum"=w1278) -> ("Props"=w1286:T19)  [unwired: 7 in, 3 out]
                n611 = Unbundle(w1286) -> ("Caption"=w1284:string, "Description"=w1283:string, "Tip Strip"=w1282:string)  [unwired: 1 out]
                n612 = Bundle By Name(cluster=w1277, "Ctl Caption"=w1284, "Ctl Description"=w1283, "Ctl Tooltip"=w1282) -> (w1285:T18)
                n613 = in-place-array #5(w1285) -> (w1272:T18[])  [unwired: 1 out]
                n614 = in-place-array #6(FALSE) -> (w1273:bool[])  [unwired: 1 out]
              }
            }
          }
        }
      }
      frame "Ctrl Props: Update" {
        n615 = Empty String/Path?(string/path=w1305) -> (empty?=w1306:bool)
        n616 = for {
          tunnel: w1315 -> [w1341] mode=indexing
          tunnel: [w1340] -> w1319 mode=indexing
          n617 = Unbundle By Name(w1341) -> ("Tree Tag"=w1340:string)
        }
        n618 = case shown="False" w1306 {
          tunnel: w1320 -> [_ w1327]
          tunnel: [w1325 w1326] -> w1302
          tunnel: w1305 -> [w1325 _]
          frame False {
          }
          frame True {
            n619 = Index Array(array=w1327) -> (element=w1326:string)  [unwired: 1 in]
          }
        }
        n620 = case shown="True" w1304 {
          tunnel: w1319 -> [_ w1324]
          tunnel: [-1 ("index of element") w1323] -> w1308
          tunnel: w1302 -> [_ w1322]
          frame False {
          }
          frame True {
            n621 = Search 1D Array(1D array=w1324, element=w1322) -> (index of element=w1323:i32)  [unwired: 1 in]
          }
        }
        n622 = case shown="0.." w1308 {
          selector: w1308 -> [_ w1333]
          tunnel: w1315 -> [_ w1339]
          tunnel: [_ w1337] -> w1313
          tunnel: [_ w1336] -> w1312
          tunnel: [_ w1335] -> w1311
          tunnel: [_ w1334] -> w1310
          tunnel: [w1328 _] -> w1303
          tunnel: [w1328 T10."Disabled" ("Disabled")] -> w1298
          tunnel: [_ w1329] -> w1297
          frame ..-1 {
            w1328 = T10."Disabled and Grayed Out" ("Disabled")
          }
          frame 0.. {
            n623 = Index Array(array=w1339, index=w1333) -> (element=w1338:T18)
            n624 = Unbundle By Name(w1338) -> ("Control Label"=w1337:string, "Page Refnum"=w1331:refnum<vi>, "Ctl Caption"=w1336:string, "Ctl Description"=w1335:string, "Ctl Tooltip"=w1334:string)
            n625 = Not A Number/Path/Refnum?(number/path/refnum=w1331) -> (NaN/Path/Refnum?=w1330:bool)
            n626 = Not(x=w1330) -> (.not. x?=w1329:bool)
          }
        }
        "Ctrl Label" <- w1313
        n627 = property on="Ctrl Tree" class="Tree (strict)"("Active Item Tag"=w1302) -> ("Glyph"=w1301:i32)  [unwired: 2 in, 2 out]
        n628 = invoke on="Ctrl Tree" class="Tree (strict)" method="Custom Item Symbols.Get Symbol"("index"=w1301) -> ("Custom Glyphs:Get Glyph"=w1300:T6)  [unwired: 3 in, 3 out]
        n629 = property on="Ctrl Label" class="Str"("DisabledEnum"=w1298) -> ()  [unwired: 2 in, 2 out]
        n630 = property on="Ctrl Description" class="Str"("Value"=w1311, "DisabledEnum"=w1303) -> ()  [unwired: 2 in, 2 out]
        n631 = property on="Ctrl Tooltip" class="Str"("Value"=w1310, "DisabledEnum"=w1303) -> ()  [unwired: 2 in, 2 out]
        n632 = call <vilib>:"Draw Flattened Pixmap.vi"("image data"=w1300) -> ("new picture"=→"Ctrl Icon":picture)  [unwired: 8 in]
        n633 = Concatenate Strings(w1318) -> (w1309:string)
        n634 = Select(t="Page Caption", s=w1297, f="Caption") -> (s? t:f=w1294:string)
        n635 = property on="Ctrl Caption" class="Str"("Caption.Text"=w1294, "Value"=w1312, "DisabledEnum"=w1303) -> ()  [unwired: 2 in, 2 out]
      }
      frame "Ctrl Props: Apply" {
        n636 = for {
          tunnel: w1350 -> [w1361] mode=indexing
          tunnel: [w1360] -> w1354 mode=indexing
          n637 = Unbundle By Name(w1361) -> ("Tree Tag"=w1360:string)
        }
        n638 = Search 1D Array(1D array=w1354, element=w1342) -> (index of element=w1349:i32)  [unwired: 1 in]
        n639 = in-place {
          n640 = in-place-array #7(w1350, w1349) -> (w1356:T18)
          n641 = in-place {
            n642 = in-place-cluster #8(w1356) -> ()  [unwired: 3 out]
            n643 = in-place-cluster #8("Ctl Caption"="Ctrl Caption", "Ctl Description"="Ctrl Description", "Ctl Tooltip"="Ctrl Tooltip") -> (w1355:T18)
          }
          n644 = in-place-array #7(w1355) -> (w1348:T18[])  [unwired: 1 out]
        }
        n645 = Format Into String(format string="Defer FP Update = ON;\n\nCtrl Props: Update = %s;\nTree: Update Info = %s;\nControl Appearance;\n\nDefer FP Update = OFF;", w1342, w1342) -> (resulting string=w1343:string)  [unwired: 2 in, 1 out]
        n646 = Concatenate Strings(w1343, w1347) -> (w1346:string)
      }
      frame "--------------------------------------- 7" {
      }
      frame "Apply to VI" {
        n647 = Unbundle By Name(w1384) -> ("VI Reference"=w1373:refnum<vi>)
        n648 = call <vilib>:"Clear Errors.vi"() -> ("error out"=w1385:errorcluster)  [unwired: 6 in, 1 out]
        n649 = invoke class="VI" method="Transaction.Begin Undo"(reference=w1373, "Name"="Changes by VIDocEditor") -> (reference out=w1371:refnum<vi>)  [unwired: 2 in, 3 out]
        n650 = for {
          N: 10 -> [_]
          tunnel: w1371 -> [w1425]
          tunnel: w1384 -> [w1424]
          shift-right: [w1423] -> w1383
          shift-left: w1385 -> [w1422]
          i -> [w1426]
          n651 = case shown="6" w1426 {
            tunnel: w1425 -> [_ w1436 w1451 w1465 w1479 w1493 w1504 w1517 w1531]
            tunnel: w1424 -> [_ w1435 w1450 w1464 w1478 w1492 w1507 w1520 w1534]
            tunnel: [w1427 w1429 w1445 w1459 w1473 w1487 w1505 w1513 w1527] -> w1423
            tunnel: w1422 -> [w1427 w1428 w1444 w1457 w1471 w1485 w1503 w1513 w1527]
            frame Default {
            }
            frame 0 {
              n652 = Unbundle By Name(w1435) -> ("Description"=w1431:string)
              n653 = property class="VI"(reference=w1436, error in=w1428) -> (reference out=w1432:refnum<vi>, error out=w1430:errorcluster, "Description"=w1434:string)
              n654 = Not Equal?(x=w1434, y=w1431) -> (x != y?=w1433:bool)
              n655 = case shown="True" w1433 {
                tunnel: w1432 -> [_ w1441]
                tunnel: w1431 -> [_ w1440]
                tunnel: w1430 -> [w1437 w1439]
                tunnel: [w1437 w1438] -> w1429
                frame False {
                }
                frame True {
                  n656 = property class="VI"(reference=w1441, error in=w1439, "Description"=w1440) -> (error out=w1438:errorcluster)  [unwired: 1 out]
                }
              }
            }
            frame 1 {
              n657 = property class="VI"(reference=w1451, error in=w1444) -> (reference out=w1448:refnum<vi>, error out=w1446:errorcluster, "Help.Path"=w1443:path)
              n658 = Unbundle By Name(w1450) -> ("Help.Path"=w1447:path)
              n659 = call "VIH - VI Doc Editor - Adjust Path.vi"("Path"=w1443) -> ("Path out"=w1442:path)  [unwired: 10 in]
              n660 = Not Equal?(x=w1442, y=w1447) -> (x != y?=w1449:bool)
              n661 = case shown="True" w1449 {
                tunnel: w1448 -> [_ w1456]
                tunnel: w1447 -> [_ w1455]
                tunnel: w1446 -> [w1452 w1454]
                tunnel: [w1452 w1453] -> w1445
                frame False {
                }
                frame True {
                  n662 = property class="VI"(reference=w1456, error in=w1454, "Help.Path"=w1455) -> (error out=w1453:errorcluster)  [unwired: 1 out]
                }
              }
            }
            frame 2 {
              n663 = Unbundle By Name(w1464) -> ("Help.Tag"=w1461:string)
              n664 = property class="VI"(reference=w1465, error in=w1457) -> (reference out=w1462:refnum<vi>, error out=w1460:errorcluster, "Help.Tag"=w1458:string)
              n665 = Not Equal?(x=w1458, y=w1461) -> (x != y?=w1463:bool)
              n666 = case shown="True" w1463 {
                tunnel: w1462 -> [_ w1470]
                tunnel: w1461 -> [_ w1469]
                tunnel: w1460 -> [w1466 w1468]
                tunnel: [w1466 w1467] -> w1459
                frame False {
                }
                frame True {
                  n667 = property class="VI"(reference=w1470, error in=w1468, "Help.Tag"=w1469) -> (error out=w1467:errorcluster)  [unwired: 1 out]
                }
              }
            }
            frame 3 {
              n668 = property class="VI"(reference=w1479, error in=w1471) -> (reference out=w1476:refnum<vi>, error out=w1474:errorcluster, "Front Panel.CustomTitle"=w1472:bool)
              n669 = Unbundle By Name(w1478) -> ("CustomTitle"=w1475:bool)
              n670 = Not Equal?(x=w1472, y=w1475) -> (x != y?=w1477:bool)
              n671 = case shown="True" w1477 {
                tunnel: w1476 -> [_ w1484]
                tunnel: w1475 -> [_ w1483]
                tunnel: w1474 -> [w1480 w1482]
                tunnel: [w1480 w1481] -> w1473
                frame False {
                }
                frame True {
                  n672 = property class="VI"(reference=w1484, error in=w1482, "Front Panel.CustomTitle"=w1483) -> (error out=w1481:errorcluster)  [unwired: 1 out]
                }
              }
            }
            frame 4 {
              n673 = property class="VI"(reference=w1493, error in=w1485) -> (reference out=w1490:refnum<vi>, error out=w1488:errorcluster, "Front Panel.Title"=w1486:string)
              n674 = Unbundle By Name(w1492) -> ("Title"=w1489:string)
              n675 = Not Equal?(x=w1486, y=w1489) -> (x != y?=w1491:bool)
              n676 = case shown="True" w1491 {
                tunnel: w1490 -> [_ w1498]
                tunnel: w1489 -> [_ w1497]
                tunnel: w1488 -> [w1494 w1496]
                tunnel: [w1494 w1495] -> w1487
                frame False {
                }
                frame True {
                  n677 = property class="VI"(reference=w1498, error in=w1496, "Front Panel.Title"=w1497) -> (error out=w1495:errorcluster)  [unwired: 1 out]
                }
              }
            }
            frame 5 {
              n678 = invoke class="VI" method="VI Icon.Get as Image Data"(reference=w1504, error in=w1503) -> (reference out=w1502:refnum<vi>, error out=w1501:errorcluster, "ImageData"=w1499:T6)  [unwired: 4 in, 3 out]
              n679 = Unbundle By Name(w1507) -> ("Icon"=w1500:T6)
              n680 = Not Equal?(x=w1499, y=w1500) -> (x != y?=w1506:bool)
              n681 = case shown="True" w1506 {
                tunnel: w1502 -> [_ w1512]
                tunnel: w1501 -> [w1508 w1511]
                tunnel: [w1508 w1510] -> w1505
                tunnel: w1500 -> [_ w1509]
                frame False {
                }
                frame True {
                  n682 = invoke class="VI" method="VI Icon.Set from Image Data"(reference=w1512, error in=w1511, "ImageData"=w1509) -> (error out=w1510:errorcluster)  [unwired: 3 in, 5 out]
                }
              }
            }
            frame 6 {
              n683 = Unbundle By Name(w1520) -> ("Help.UseWebUrl"=w1518:bool)
              n684 = call "VIH Platform - LabVIEW - VI Property - Help - Use Web Url (2014).vi"("error in"=w1513, "VI Refnum"=w1517) -> ("error out"=w1514:errorcluster, "UseWebURL out"=w1515:bool, "dup VI Refnum"=w1516:refnum<vi>)  [unwired: 7 in]
              n685 = Not Equal?(x=w1515, y=w1518) -> (x != y?=w1519:bool)
              n686 = case shown="True" w1519 {
                tunnel: w1516 -> [_ w1526]
                tunnel: w1518 -> [_ w1525]
                tunnel: [w1521 w1523] -> _
                tunnel: w1514 -> [w1521 w1524]
                frame False {
                }
                frame True {
                  n687 = call "VIH Platform - LabVIEW - VI Property - Help - Use Web Url (2014).vi"("cmd (read)"=enum16{"read", "write"}."write", "error in"=w1524, "UseWebURL"=w1525, "VI Refnum"=w1526) -> ("error out"=w1523:errorcluster)  [unwired: 5 in, 2 out]
                }
              }
            }
            frame 7 {
              n688 = Unbundle By Name(w1534) -> ("Help.WebUrl"=w1532:string)
              n689 = call "VIH Platform - LabVIEW - VI Property - Help - Web Url (2014).vi"("error in"=w1527, "VI Refnum"=w1531) -> ("error out"=w1528:errorcluster, "WebURL out"=w1529:string, "dup VI Refnum"=w1530:refnum<vi>)  [unwired: 7 in]
              n690 = Not Equal?(x=w1529, y=w1532) -> (x != y?=w1533:bool)
              n691 = case shown="True" w1533 {
                tunnel: w1530 -> [_ w1540]
                tunnel: w1532 -> [_ w1536]
                tunnel: [w1535 w1538] -> _
                tunnel: w1528 -> [w1535 w1539]
                frame False {
                }
                frame True {
                  n692 = call "VIH Platform - LabVIEW - VI Property - Help - Web Url (2014).vi"("cmd (read)"=enum16{"read", "write"}."write", "error in"=w1539, "WebURL"=w1536, "VI Refnum"=w1540) -> ("error out"=w1538:errorcluster)  [unwired: 5 in, 2 out]
                }
              }
            }
          }
        }
        n693 = for {
          shift-right: [w1407] -> w1369
          shift-left: w1383 -> [w1408]
          tunnel: w1382 -> [w1409] mode=indexing
          tunnel: w1381 -> [w1406] mode=indexing
          n694 = case shown="True" w1406 {
            tunnel: w1409 -> [_ w1421]
            tunnel: w1408 -> [w1410 w1420]
            tunnel: [w1410 w1419] -> w1407
            frame False {
            }
            frame True {
              n695 = Unbundle By Name(w1421) -> ("Page Refnum"=w1411:refnum<vi>, "Ctl Refnum"=w1414:refnum<vi>, "Ctl Caption"=w1418:string, "Ctl Description"=w1417:string, "Ctl Tooltip"=w1416:string)
              n696 = Not A Number/Path/Refnum?(number/path/refnum=w1414) -> (NaN/Path/Refnum?=w1413:bool)
              n697 = Select(t=w1411, s=w1413, f=w1414) -> (s? t:f=w1412:refnum<vi>)
              n698 = Bundle("Ctl Caption"=w1418, "Ctl Description"=w1417, "Ctl Tooltip"=w1416) -> (w1415:T25)  [unwired: 1 in]
              n699 = call "VIH - VI Doc Editor #2 - GenObject Properties - Write.vi"("error in"=w1420, "Props"=w1415, "Ctrl Refnum"=w1412) -> ("error out"=w1419:errorcluster)  [unwired: 7 in, 1 out]
            }
          }
        }
        n700 = call <vilib>:"Clear Errors.vi"("error in (no error)"=w1369) -> ("error out"=w1368:errorcluster)  [unwired: 5 in, 1 out]
        n701 = invoke class="VI" method="Transaction.End Undo"(reference=w1371, error in=w1368) -> (reference out=w1370:refnum<vi>)  [unwired: 1 in, 2 out]
        n702 = property on="VI Version" class="Str"() -> ("Text.FontColor"=w1376:u32)  [unwired: 2 in, 2 out]
        n703 = Equal?(x=w1376, y=u32 16711680) -> (x = y?=w1374:bool)
        n704 = case shown="\"SAVE\"" w1380 {
          tunnel: w1369 -> [w1390 w1396]
          tunnel: w1370 -> [_ w1395]
          tunnel: [w1390 w1394] -> w1379
          tunnel: w1374 -> [_ w1393]
          frame Default {
          }
          frame "SAVE" {
            n705 = case shown="True" w1393 {
              tunnel: [TRUE w1401] -> w1392
              tunnel: "The VI was last saved with a different version of LabVIEW. Are you sure to save the VI with the current LabVIEW version?" -> [_ w1398]
              frame False {
              }
              frame True {
                n706 = Two Button Dialog(message=w1398, 1:"No ", 2:"Yes") -> (T button?=w1401:bool)
              }
            }
            n707 = case shown="True" w1392 {
              tunnel: w1396 -> [w1402 w1405]
              tunnel: w1395 -> [_ w1404]
              tunnel: [w1402 w1403] -> w1394
              frame False {
              }
              frame True {
                n708 = invoke class="VI" method="Save.Instrument"(reference=w1404, error in=w1405) -> (error out=w1403:errorcluster)  [unwired: 4 in, 5 out]
              }
            }
          }
        }
        n709 = Concatenate Strings("Set Busy = ON;\nDefer FP Update = ON;\n\nVI Props: Update;\nUpdate VI Conpane Image;\nVI Props: Changed?;\n\nCtrl Props: Update;\nTree: Update Info = ALL;\n\nControl Appearance;\n\nDefer FP Update = OFF;\nSet Busy = OFF;", w1389) -> (w1378:string)
        n710 = call <vilib>:"Simple Error Handler.vi"("error in (no error)"=w1379) -> ()  [unwired: 4 in, 5 out]
      }
      frame "Restore VI Properties" {
        n711 = Match Pattern(string=w1547, regular expression="\\?") -> (before substring=w1544:string, after substring=w1545:string)  [unwired: 1 in, 2 out]
        n712 = call <vilib>:"Trim Whitespace.vi"("string"=w1544) -> ("trimmed string"=w1543:string)  [unwired: 1 in]
        n713 = call <vilib>:"Trim Whitespace.vi"("string"=w1545) -> ("trimmed string"=w1541:string)  [unwired: 1 in]
        n714 = case shown="\"CTRL\"" w1543 {
          tunnel: "Set Busy = ON;\nDefer FP Update = ON;\n\nVI Props: Read From VI;\nVI Props: Update;\n\nVI Props: Changed?;\n#= Update VI Conpane Image;\n\nControl Appearance;\n\nDefer FP Update = OFF;\nSet Busy = OFF;" -> [_ w1557 w1561 _]
          tunnel: [_ w1557 w1560 w1564] -> w1548
          tunnel: "Set Busy = ON;\nDefer FP Update = ON;\n\nCtrl Props: Read From VI = %s;\nCtrl Props: Update;\n\nTree: Update Info = %s;\n\nControl Appearance;\n\nDefer FP Update = OFF;\nSet Busy = OFF;" -> [_ _ w1559 w1563]
          tunnel: w1541 -> [_ _ _ w1562]
          frame Default {
            n715 = call <vilib>:"Beep.vi"() -> ()  [unwired: 12 in]
          }
          frame "VI" {
          }
          frame "ALL" {
            w1558 = "ALL"
            n716 = Format Into String(format string=w1559, initial string=w1561, w1558, w1558) -> (resulting string=w1560:string)  [unwired: 1 in, 1 out]
          }
          frame "CTRL" {
            n717 = Format Into String(format string=w1563, w1562, w1562) -> (resulting string=w1564:string)  [unwired: 2 in, 1 out]
          }
        }
        n718 = Concatenate Strings(w1548, w1556) -> (w1550:string)
      }
    }
  }
